vi "Trajectory Builder.vi"() -> ()   [LabVIEW 2023]
uses:
  Types/Limits.ctl
  Types/Overrides.ctl
  Types/Trajectory Data.ctl
  Types/Segment Type.ctl
  Types/Path Type.ctl
  Types/Drive Type.ctl
  Types/Angluar Limits.ctl
  Types/Command Editor Info.ctl
  Types/Single Cmd Info.ctl
  <vilib>/picture/picture.llb/imagedata.ctl
  <vilib>/Utility/miscctls.llb/LVPositionTypeDef.ctl
  <vilib>/Utility/miscctls.llb/LVRowAndColumnTypeDef.ctl
  Types/Internal Path Stuff.ctl
  <vilib>/event_ctls.llb/lveventtype.ctl
  6a65ebb4-e776-4ba2-b94f-6ff829af6114.vi
  6a65ebb4-e776-4ba2-b94f-6ff829af6114.vi/c0db33a9-eb6c-44d9-b982-8563e05d2734.vi
  6a65ebb4-e776-4ba2-b94f-6ff829af6114.vi/ae3535a8-0066-4e8d-a5de-b07ac05a7c65.vi
  6a65ebb4-e776-4ba2-b94f-6ff829af6114.vi/dda8e586-731b-4197-ad83-6a4d05585a0a.vi
  Global Settings.vi
  <vilib>/Utility/cursorutil.llb/Set Cursor (Icon Pict).vi
  <vilib>/Comparison/Less/Less Functor/Less Functor.lvclass
panel:
  in  "Delete":bool
  in  "New Page Selector":T1(radio)
  in  "Push":bool
  out "Picture":picture
  out "RS":bool=TRUE
  in  "Cache":T5
  in  "Zero Velocity":bool
  in  "Reverse Path":bool
  in  "Robot Backwards":bool
  out "Duration (s)":dbl format="%#.4g"
  out "Distance (ft)":dbl format="%#.1g"
  in  "Instructions":string="Directions:\nUse mouse to ...\n    move robot position (rectangle with arrow)\n    rotate robot (red arrow)\n    move waypoints (numbered circles)\nClick in open space to add a waypoint\nShift click to delete a waypoint\nHover over a waypoint and use arrow keys to nudge\n\nTime slider and Play button will run robot along path to test for collisions.\n\nNew creates a new path at default location\n\nAppend creates a path using current path's position and heading.\n\nTo add a command, move robot using Time slider and double click the Command in Palette.\n\nYou can modify command timing in the graph or Command Sequencer tree.\n\nEnable/disable a command by clicking on the enable column item.\n\nDelete a command by shift-clicking in the enable column.\n\nTo configure command parameters, Select the command name in the tree, Open Panel, enter parameters, and Inhale the parameters.\n\nYou may sometimes want to type values into WayPoints directly.\n\nOverrides allow you to set accel and V limits for any turn."
  out "Command Palette":picture
  in  "Directory":bool
  in  "Tab Control":T1(tab)
  in  "Vertical Reflection":bool
  in  "Angular Limits":T6={"Velocity (deg/s)"=6.0, "Accel (deg/s^2)"=360.0, "Jerk (deg/s^3)"=1000.0} {"Jerk (deg/s^3)" min=0.01 step=1.0; "Accel (deg/s^2)" min=0.01; "Velocity (deg/s)" min=0.01}
  in  "Path Type":T7=enum."Bezier"
  in  "Overrides":T8=[{"Count"="1", "Angular Override"=0.0, "Enabled?"=FALSE, "Velocity Override"=6.0, "Angle Override"=nan}] {"Angle Override" step=5.0; "Velocity Override" step=5.0; "Angular Override" step=5.0}
  in  "Horizontal Reflection":bool
  in  "Sample Period (s)":dbl=0.02 min=0.001 max=1.0 format="%#_6p"
  in  "Limits":T9={"Velocity (fps)"=6.0, "Accel (fps^2)"=15.0, "Jerk (fps^3)"=150.0, "StoopidFast (fps)"=6.0} {"StoopidFast (fps)" min=0.01; "Jerk (fps^3)" min=0.01 step=1.0; "Accel (fps^2)" min=0.01; "Velocity (fps)" min=0.01}
  in  "Conditions":T10 {"vFinal (fps)" min=0.0; "vInitial (fps)" min=0.0}
  in  "Drive Type":T11
  in  "Turn Rate":dbl=5.0 format="%#_13g"
  in  "WayPoints":cluster{"x":dbl, "y":dbl, "th":dbl}[](array[cluster])
  in  "Turn Angle Limit (deg)":dbl=90.0
  in  "Allow Angles > 90":bool=TRUE
  in  "Stoopid Overlap %":dbl min=0.0
  in  "Unjank":bool
  in  "Turn Deceleration":bool=TRUE
  in  "Turn Acceleration":bool=TRUE
  out "Trajectory Data":T12
  in  "Open Command":bool
  in  "Inhale":bool
  in  "Command Sequence":string(tree)
  in  "Projects":u16(ring) items=["Reefscape.lvproj"]
  in  "Refresh":bool
  in  "Snap to foot":bool
  in  "Angle Limiter":enum16{"90", "45", "15", "1"}(ring)=enum."15"
  in  "Snap robot to baseline":bool
  in  "Background":u16(ring) items=["RS Field"]
  in  "Robot Color":u32(colorbox)=14421504
  out "Field Size (ft)":cluster{"width":dbl, "height":dbl}={"width"=26.4166, "height"=57.5729} {"width" format="%#.1g"; "height" format="%#.1g"}
  in  "Robot Size (in)":cluster{"width":dbl, "height":dbl}={"width"=37.0, "height"=32.0}
  in  "Hide Path":bool
  in  "Time (s)":dbl(slide) scale=0.0..3.9399999119341373 scale format="%#.1g"
  in  "Play":bool
  out "fps":dbl[](graph)
  in  "Append":bool
  in  "Open":i32[](listbox)
  in  "Filename":string
  in  "Save":bool
  in  "New":bool
  # "Command Palette"
  # "StupidFast makes each linear segment into a\nvelocity ramp to max speed (for clothoid paths only)"
  # "Nicotine"
  # "A"
  # "V"
  # "O"
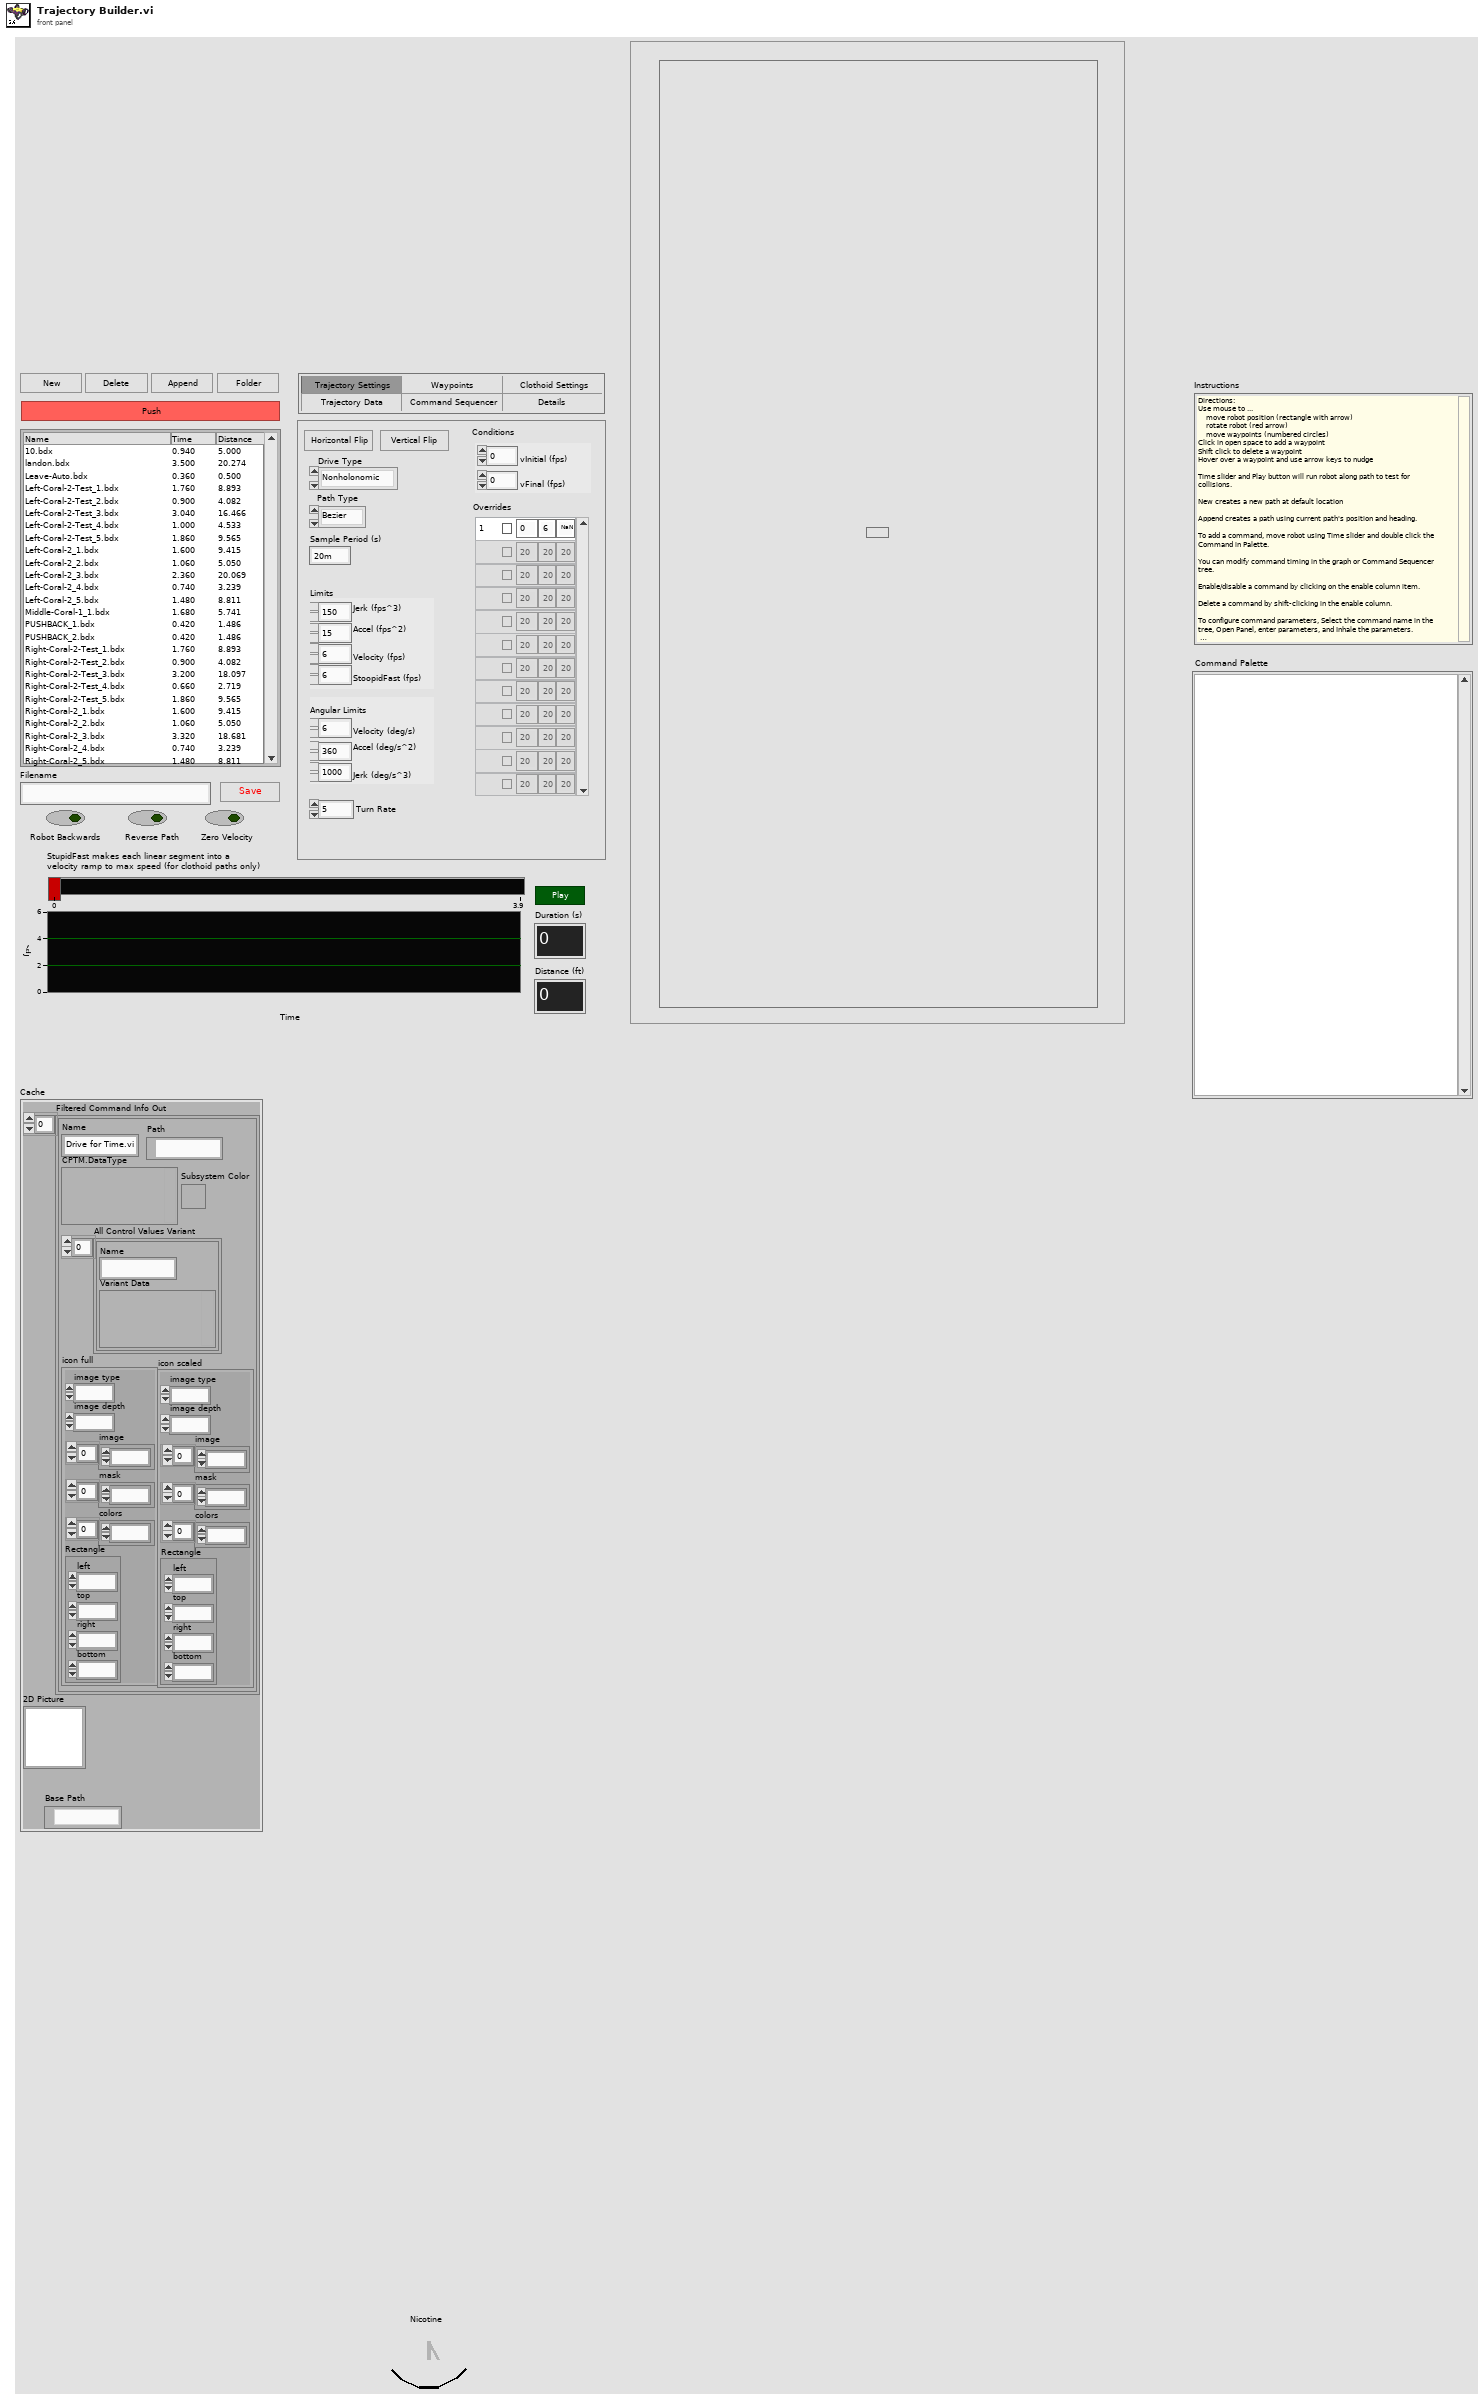
[diagram p1: front panel]
types:
  T1 = enum32{"Trajectory Settings", "Waypoints", "Clothoid Settings", "Trajectory Data", "Command Sequencer", "Details"}
  T2 = typedef "Command Editor Info.ctl" = T3[]
  T3 = typedef "Single Cmd Info.ctl" = cluster{"Name":string, "CPTM.DataType":variant, "All Control Values Variant":cluster{"Name":string, "Variant Data":variant}[], "icon full":T4, "icon scaled":T4, "Path":path, "Subsystem Color":u32}
  T4 = typedef "imagedata.ctl" = cluster{"image type":i32, "image depth":i32, "image":u8[], "mask":u8[], "colors":u32[], "Rectangle":cluster{"left":i16, "top":i16, "right":i16, "bottom":i16}}
  T5 = cluster{"Filtered Command Info Out":T2, "2D Picture":picture, "Base Path":path}
  T6 = typedef "Angluar Limits.ctl" = cluster{"Velocity (deg/s)":dbl, "Accel (deg/s^2)":dbl, "Jerk (deg/s^3)":dbl}
  T7 = typedef "Path Type.ctl" = enum16{"Clothoid", "Bezier"}
  T8 = typedef "Overrides.ctl" = cluster{"Count":string, "Angular Override":dbl, "Enabled?":bool, "Velocity Override":dbl, "Angle Override":dbl}[]
  T9 = typedef "Limits.ctl" = cluster{"Velocity (fps)":dbl, "Accel (fps^2)":dbl, "Jerk (fps^3)":dbl, "StoopidFast (fps)":dbl}
  T10 = cluster{"vInitial (fps)":dbl, "vFinal (fps)":dbl}
  T11 = typedef "Drive Type.ctl" = enum16{"Nonholonomic", "Holonomic"}
  T12 = typedef "Trajectory Data.ctl" = cluster{"Segment Name":string, "Type":T13, "Traj Pos Points":cluster{"x":dbl, "y":dbl, "th":dbl}[], "Traj Vel Points":cluster{"V":dbl, "Omega":dbl, "V vector":cluster{"y":dbl, "x":dbl}}[], "Accel Index":i32, "Decel Index":i32}[]
  T13 = typedef "Segment Type.ctl" = enum16{"Accel Straight", "Const Straight", "Blend", "Circle", "Bezier"}
  T14 = cluster{"Sample Period (s)":dbl, "Limits":T9, "Conditions":cluster{"vInitial (fps)":dbl, "vFinal (fps)":dbl}, "Overrides":T8, "Angular Limits":T6}
  T15 = typedef "LVRowAndColumnTypeDef.ctl" = cluster{"Row":i32, "Column":i32}
  T16 = typedef "LVPositionTypeDef.ctl" = cluster{"Left":i32, "Top":i32}
  T17 = cluster{"Index":i32, "Pt Test Results":enum16{"Miss", "Rect Hit", "Arrow Hit"}}
  T18 = cluster{"Drag Object":cluster{"Index":i32, "x":dbl, "y":dbl}, "Hover Object":cluster{"Index":i32, "Pt Test Results":enum16{"Miss", "Rect Hit", "Arrow Hit"}}, "Filename":string}
  T19 = cluster{"Trajectory Data":T12, "Points":cluster{"x":dbl, "y":dbl, "th":dbl}[], "output cluster":cluster{"Sample Period (s)":dbl, "Limits":T9, "Conditions":cluster{"vInitial (fps)":dbl, "vFinal (fps)":dbl}, "Overrides":T8, "Angular Limits":T6}, cluster{"Time (s)":dbl, T3, bool}[]}
  T20 = typedef "Internal Path Stuff.ctl" = cluster{"Trajectory Data":T12, "Updated Waypoints":cluster{"x":dbl, "y":dbl, "th":dbl}[], cluster{"Sample Period (s)":dbl, "Limits":T9, "Conditions":cluster{"vInitial (fps)":dbl, "vFinal (fps)":dbl}, "Overrides":T8, "Angular Limits":T6}, "Commands out":cluster{"Time (s)":dbl, T3, bool}[]}
  T21 = typedef "lveventtype.ctl" = enum32{"Null", "Timeout", "Annotation Menu Selection", "Annotation Menu Selection?", "App Instance Close", "App Instance Close?", "Autoscale Range Change", "Bookmark Info Change", "Cell Edit", "Cell Edit?", "Cursor Grab", "Cursor Grab?", "Cursor Menu Selection", "Cursor Menu Selection?", "Cursor Move", "Cursor Release", "Data Change", "Direction Change", "Display State Change", "Drag Ended", "Drag Enter", "Drag Leave", "Drag Over", "Drag Source Update", "Drag Starting", "Drag Starting?", "Drop", "Exec State Change", "Key Down", "Key Down?", "Key Repeat", "Key Repeat?", "Key Up", "Listbox Double Click", "Menu Activation?", "Menu Selection (App)", "Menu Selection? (App)", "Menu Selection (User)", "Mouse Down", "Mouse Down?", "Mouse Enter", "Mouse Leave", "Mouse Move", "Mouse Up", "Mouse Wheel", "NI Security User Change (App)", "Pane Size", "Panel Close", "Panel Close?", "Panel Resize", "Plot Attribute Change", "Scale Range Change", "Shortcut Menu Activation?", "Shortcut Menu Selection (App)", "Shortcut Menu Selection? (App)", "Shortcut Menu Selection (User)", "Tree Double Click", "Tree Drag", "Tree Drag?", "Tree Drop", "Tree Drop?", "Tree Item Close", "Tree Item Close?", "Tree Item Open", "Tree Item Open?", "User Event", "Value Change"}
  T22 = enum32{"Invalid", "Standard", "Closed", "Hidden", "Minimized", "Maximized"}
  T23 = cluster{"width":dbl, "height":dbl, "width":dbl, "height":dbl}
  T24 = cluster{"status":bool, "code":bool, "source":bool}
  T25 = cluster{"Robot Backwards":bool, "Reverse Path":bool}
  T26 = cluster{cluster{"Robot Backwards":bool, "Reverse Path":bool}, "Trajectory Data":T12, "sorted array out":cluster{"Time (s)":dbl, T3, bool}[], cluster{"Sample Period (s)":dbl, "Limits":T9, "Conditions":cluster{"vInitial (fps)":dbl, "vFinal (fps)":dbl}, "Overrides":T8, "Angular Limits":T6}, "Updated Waypoints":cluster{"x":dbl, "y":dbl, "th":dbl}[], cluster{"Time (s)":dbl, "Distance (ft)":dbl}, "Zero Velocity":bool, cluster{"Drive Type":T11, "Path Type":T7}}
  T27 = cluster{"Trajectory Data":T12, "Updated Waypoints":cluster{"x":dbl, "y":dbl, "th":dbl}[], cluster{"Sample Period (s)":dbl, "Limits":T9, "Conditions":cluster{"vInitial (fps)":dbl, "vFinal (fps)":dbl}, "Overrides":T8, "Angular Limits":T6}, "sorted array out":cluster{"Time (s)":dbl, T3, bool}[]}
  T28 = cluster{"Sample Period (s)":dbl, cluster{"Velocity (fps)":dbl, "Accel (fps^2)":dbl, "Jerk (fps^3)":dbl, "StoopidFast (fps)":dbl}, "Conditions":cluster{"vInitial (fps)":dbl, "vFinal (fps)":dbl}, "Overrides":T8, "Angular Limits":T6}
  T29 = cluster{"Velocity (fps)":dbl, "Accel (fps^2)":dbl, "Jerk (fps^3)":dbl, "StoopidFast (fps)":dbl}
  T30 = cluster{"Trajectory Data":T12, "Points out":cluster{"x":dbl, "y":dbl, "th":dbl}[], "Fields":cluster{"Sample Period (s)":dbl, cluster{"Velocity (fps)":dbl, "Accel (fps^2)":dbl, "Jerk (fps^3)":dbl, "StoopidFast (fps)":dbl}, "Conditions":cluster{"vInitial (fps)":dbl, "vFinal (fps)":dbl}, "Overrides":T8, "Angular Limits":T6}, "Commands out":cluster{"Time (s)":dbl, T3, bool}[]}
  T31 = typedef "LVPoint32TypeDef.ctl" = cluster{"Horizontal":i32, "Vertical":i32}
  T32 = cluster{"Shift":bool, "Ctrl":bool, "Alt":bool, "Cmd":bool, "Opt":bool}
  T33 = typedef "LVBoundsTypeDef.ctl" = cluster{"Width":u32, "Height":u32}
  T34 = cluster{"Snap robot to baseline":bool, "Snap to foot":bool, "Angle Limiter":enum16{"90", "45", "15", "1"}}
  T35 = cluster{i32, "Pt Test Results":enum16{"Miss", "Rect Hit", "Arrow Hit"}}
  T36 = typedef "eventvkey.ctl" = enum16{"ASCII", "Enter", "Return", "Shift", "Ctrl", "Alt", "Cmd", "Opt", "Caps", "NumLock", "Clear", "Break", "Up", "Down", "Left", "Right", "Insert", "Delete", "Home", "End", "PageUp", "PageDown", "Escape", "Help", "Pause", "ScrollLock", "F1", "F2", "F3", "F4", "F5", "F6", "F7", "F8", "F9", "F10", "F11", "F12", "F13", "F14", "F15", "F16", "F17", "F18", "F19", "F20", "F21", "F22", "F23", "F24", "Play", "VolumeUp", "VolumeDown", "Mute", "Two Byte Char"}
  T37 = cluster{"Name":string, "CPTM.DataType":variant, "Get All Control Values Variant":cluster{"Name":string, "Variant Data":variant}[], "Color 256":T4, "Subsystem Color":u32}[]
  T38 = cluster{"Filtered Command Info Out":T2, "2D Picture":picture, "stripped path":path}
  T39 = cluster{"Horizontal":dbl, "Vertical":dbl, "th":dbl}
  T40 = cluster{"Name":string, "Color":u32, "Style":i32, "Point Style":i32, "Name Visible":bool, "Allow Drag":bool, "Annotation Mode":i32, "Plot":i32, "Index":i32, "Position":cluster{"X":dbl, "Y":dbl}, "X Scale":i32, "Y Scale":u32, "Show Arrow":bool, "Lock Name":bool, "Plot Area":i32, "Label Offset":cluster{"X":dbl, "Y":dbl}}[]
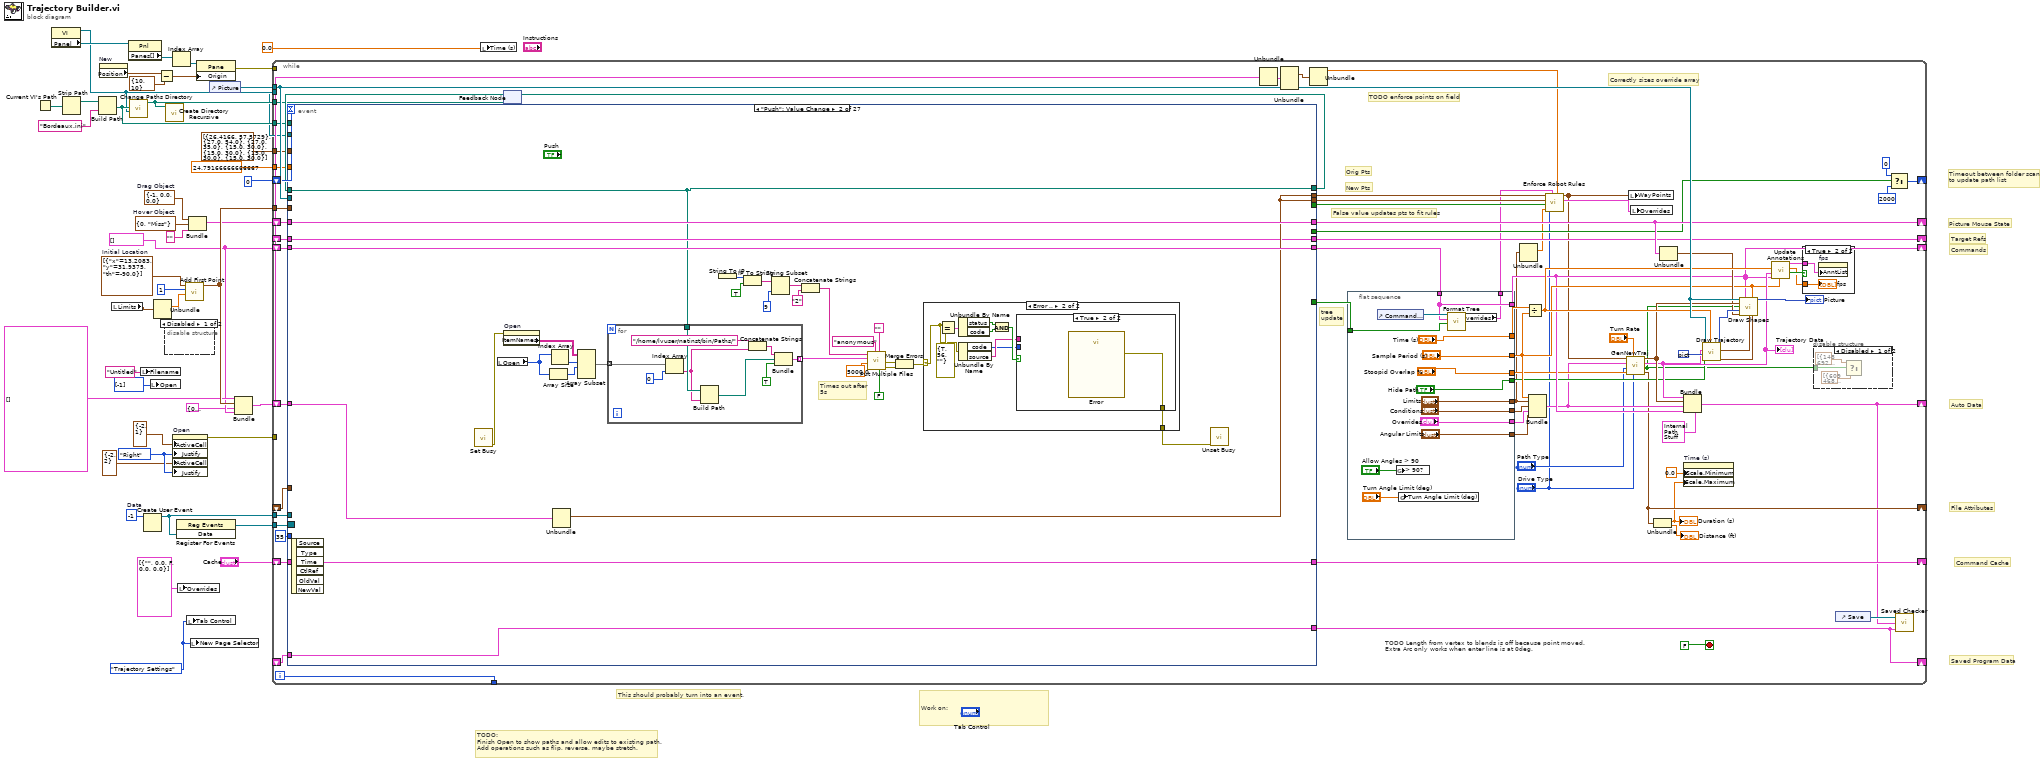
[diagram p0: block diagram]
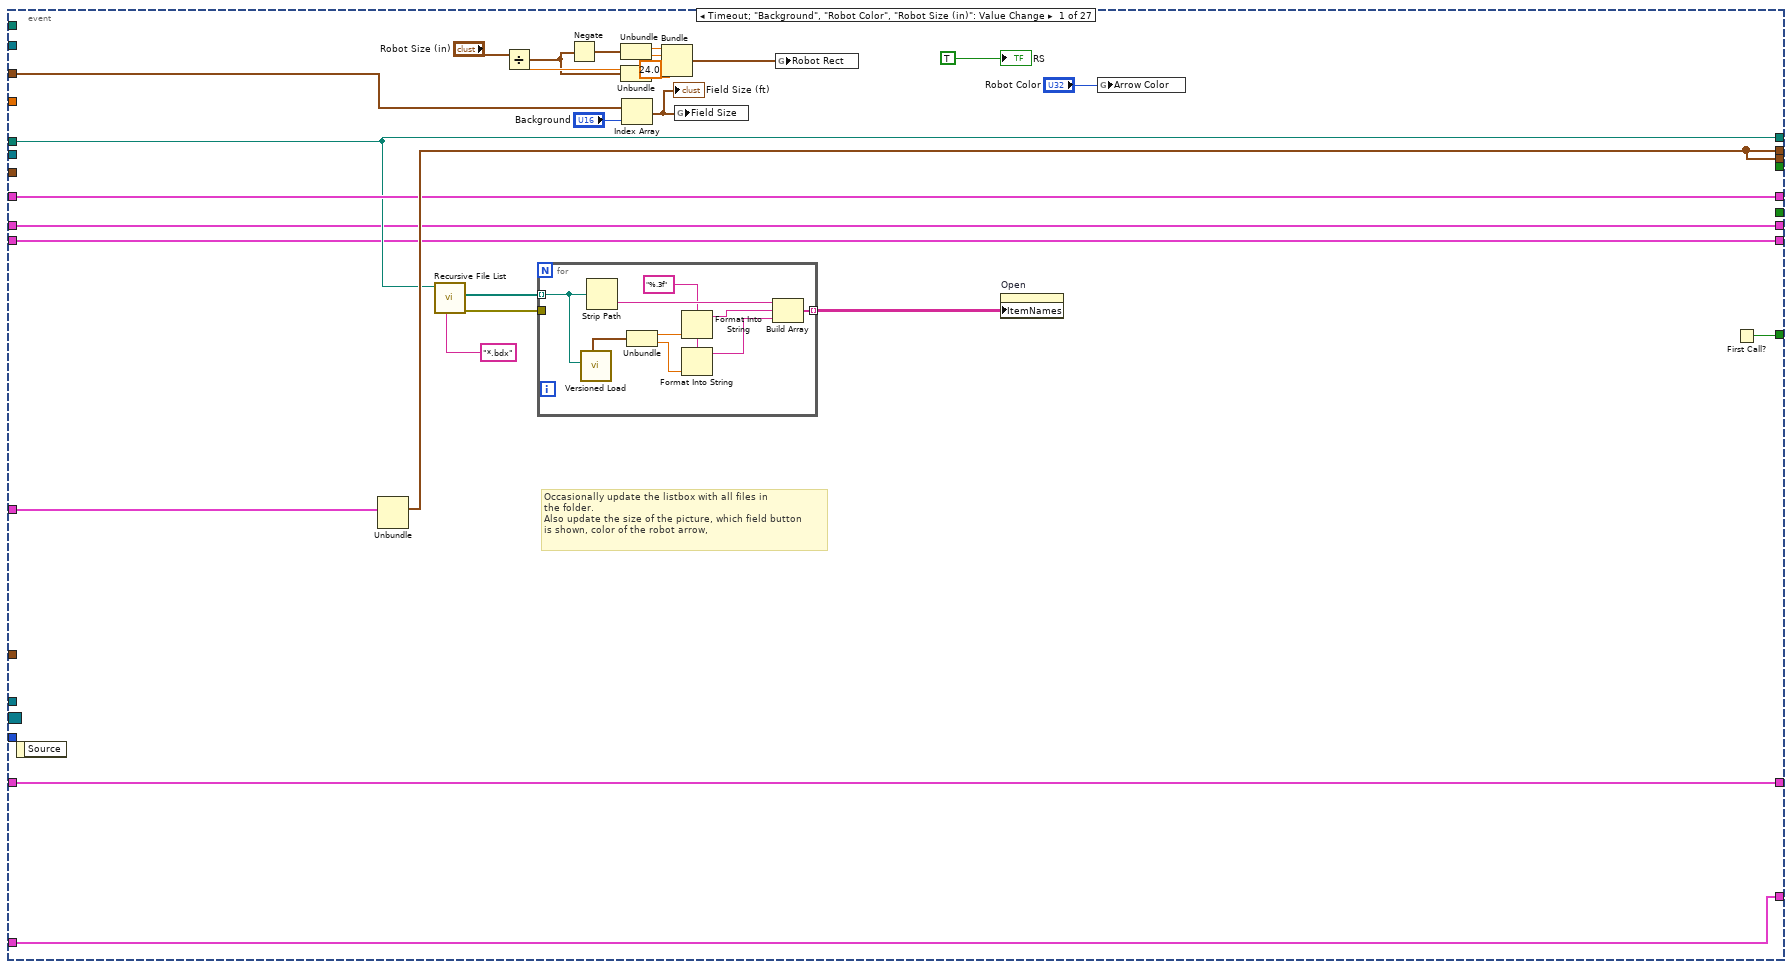
[diagram p4: hidden frame]
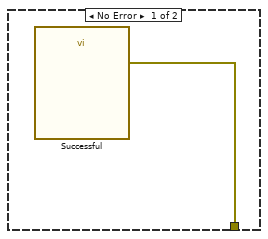
[diagram p5: hidden frame]
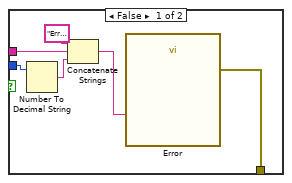
[diagram p6: hidden frame]
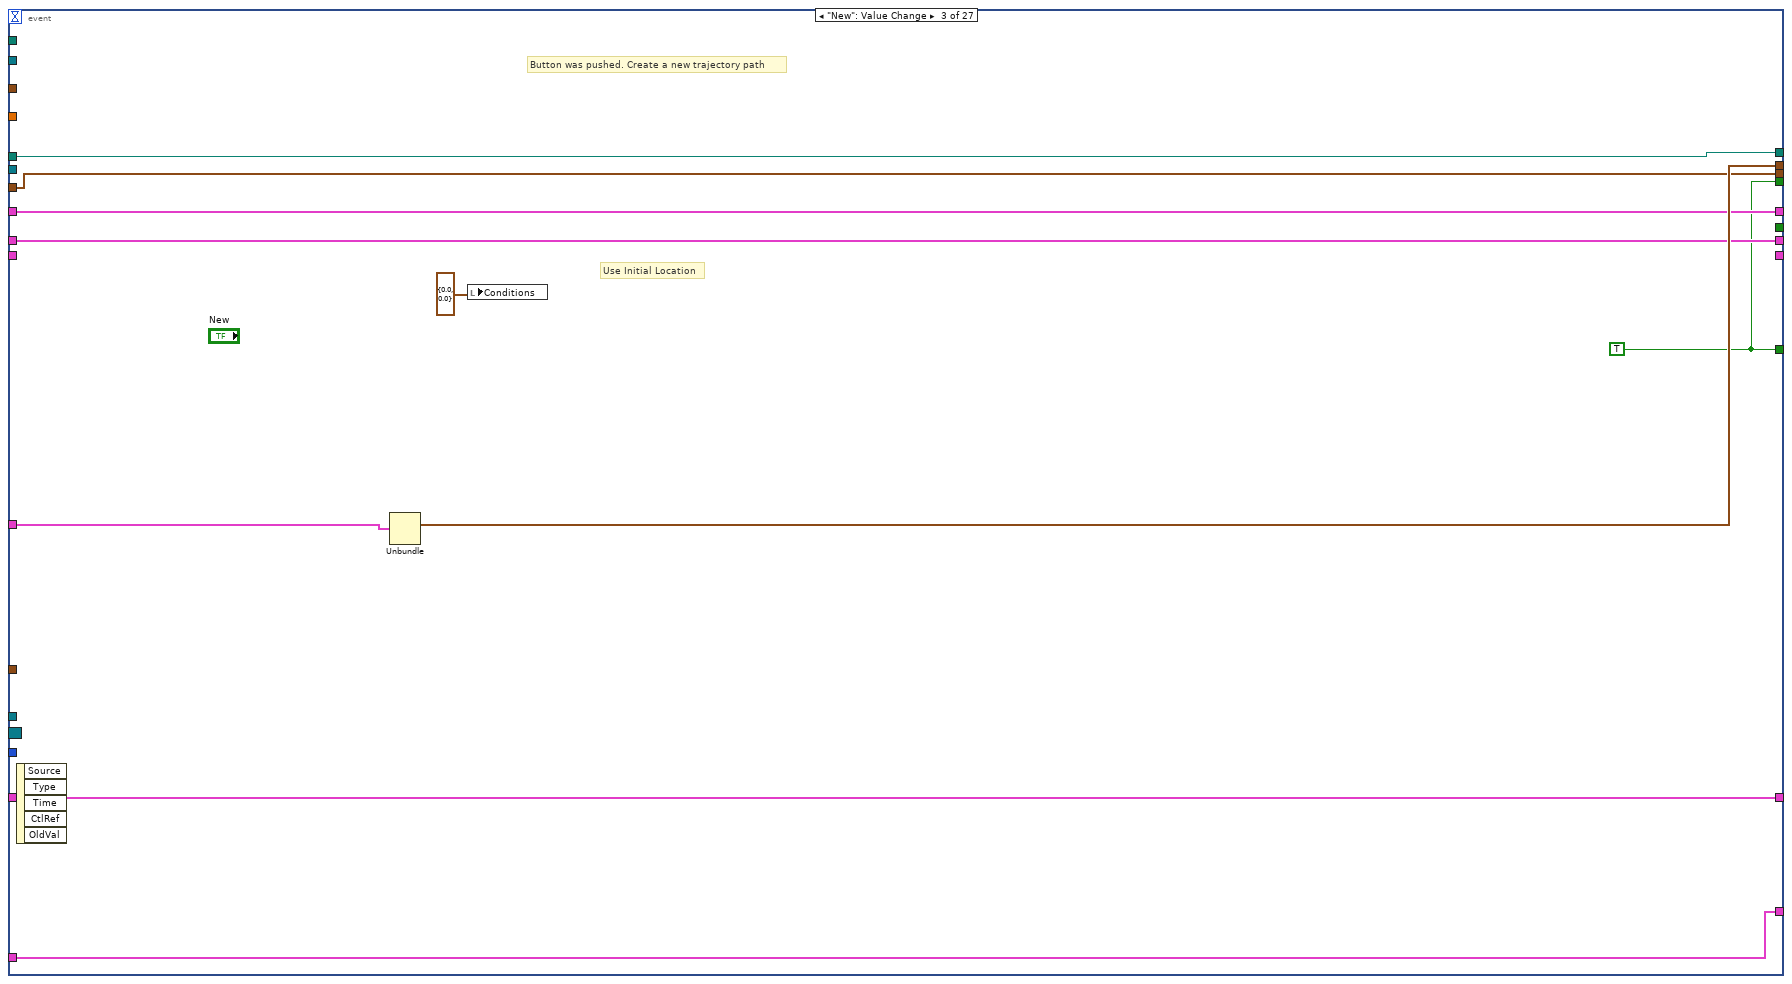
[diagram p7: hidden frame]
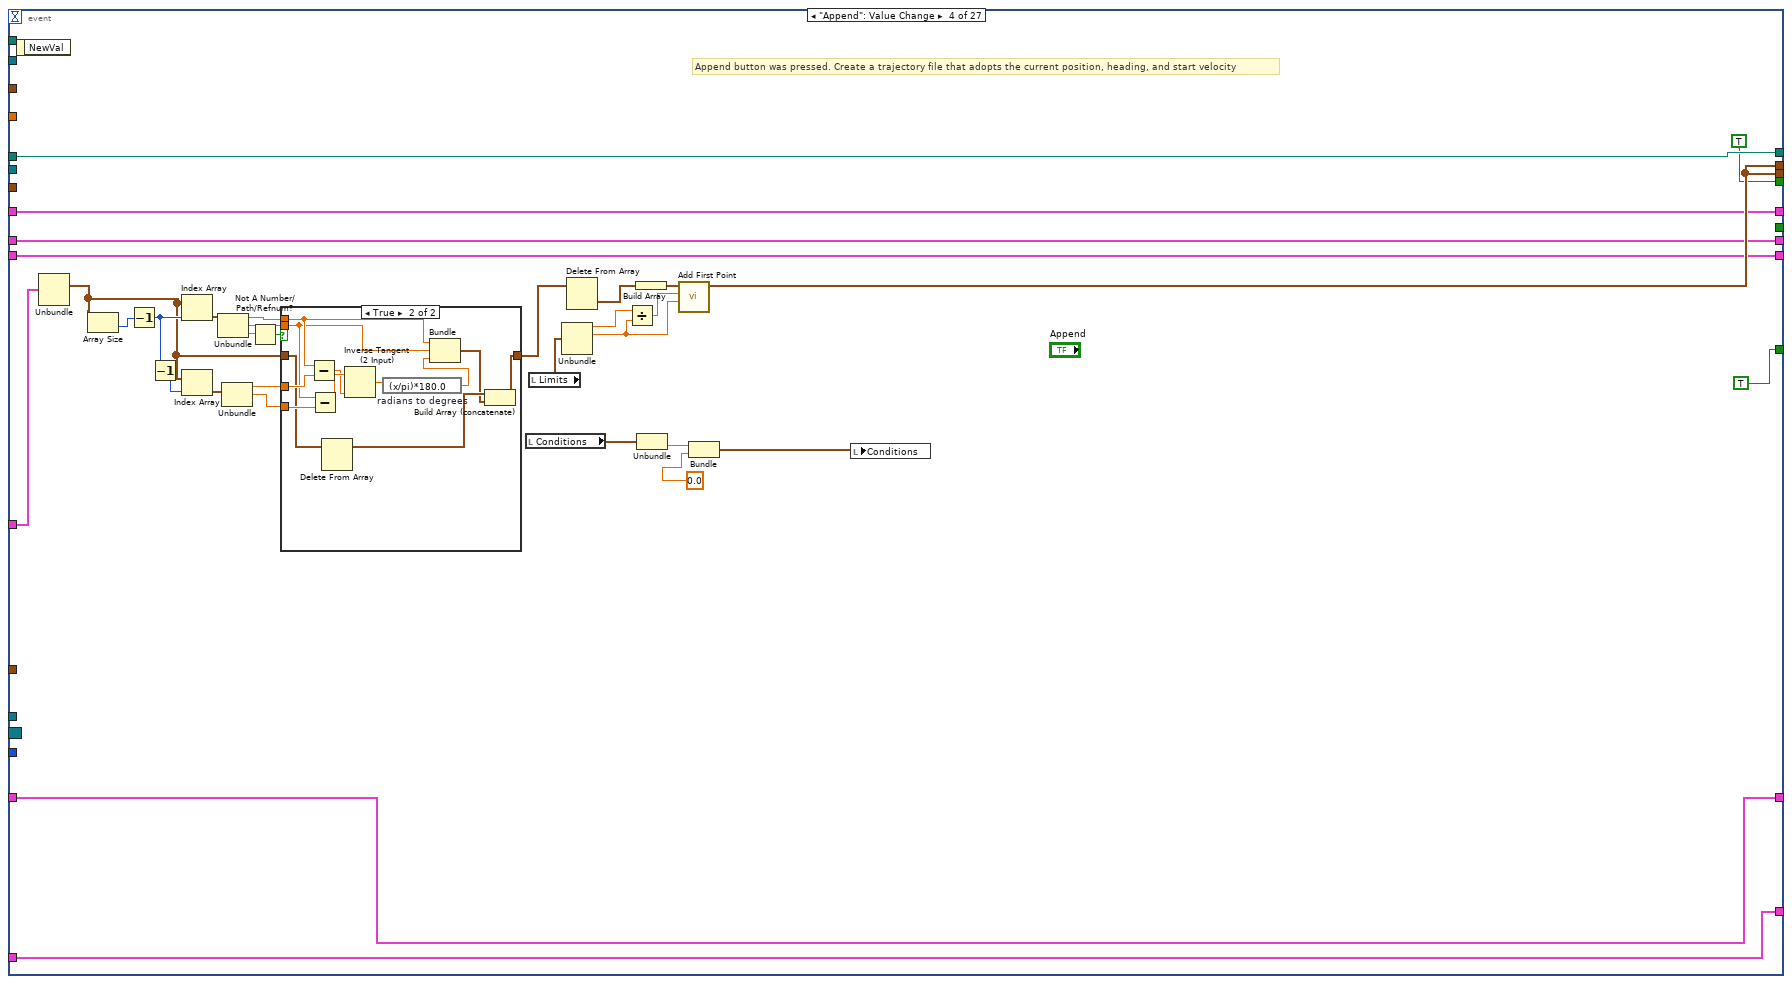
[diagram p8: hidden frame]
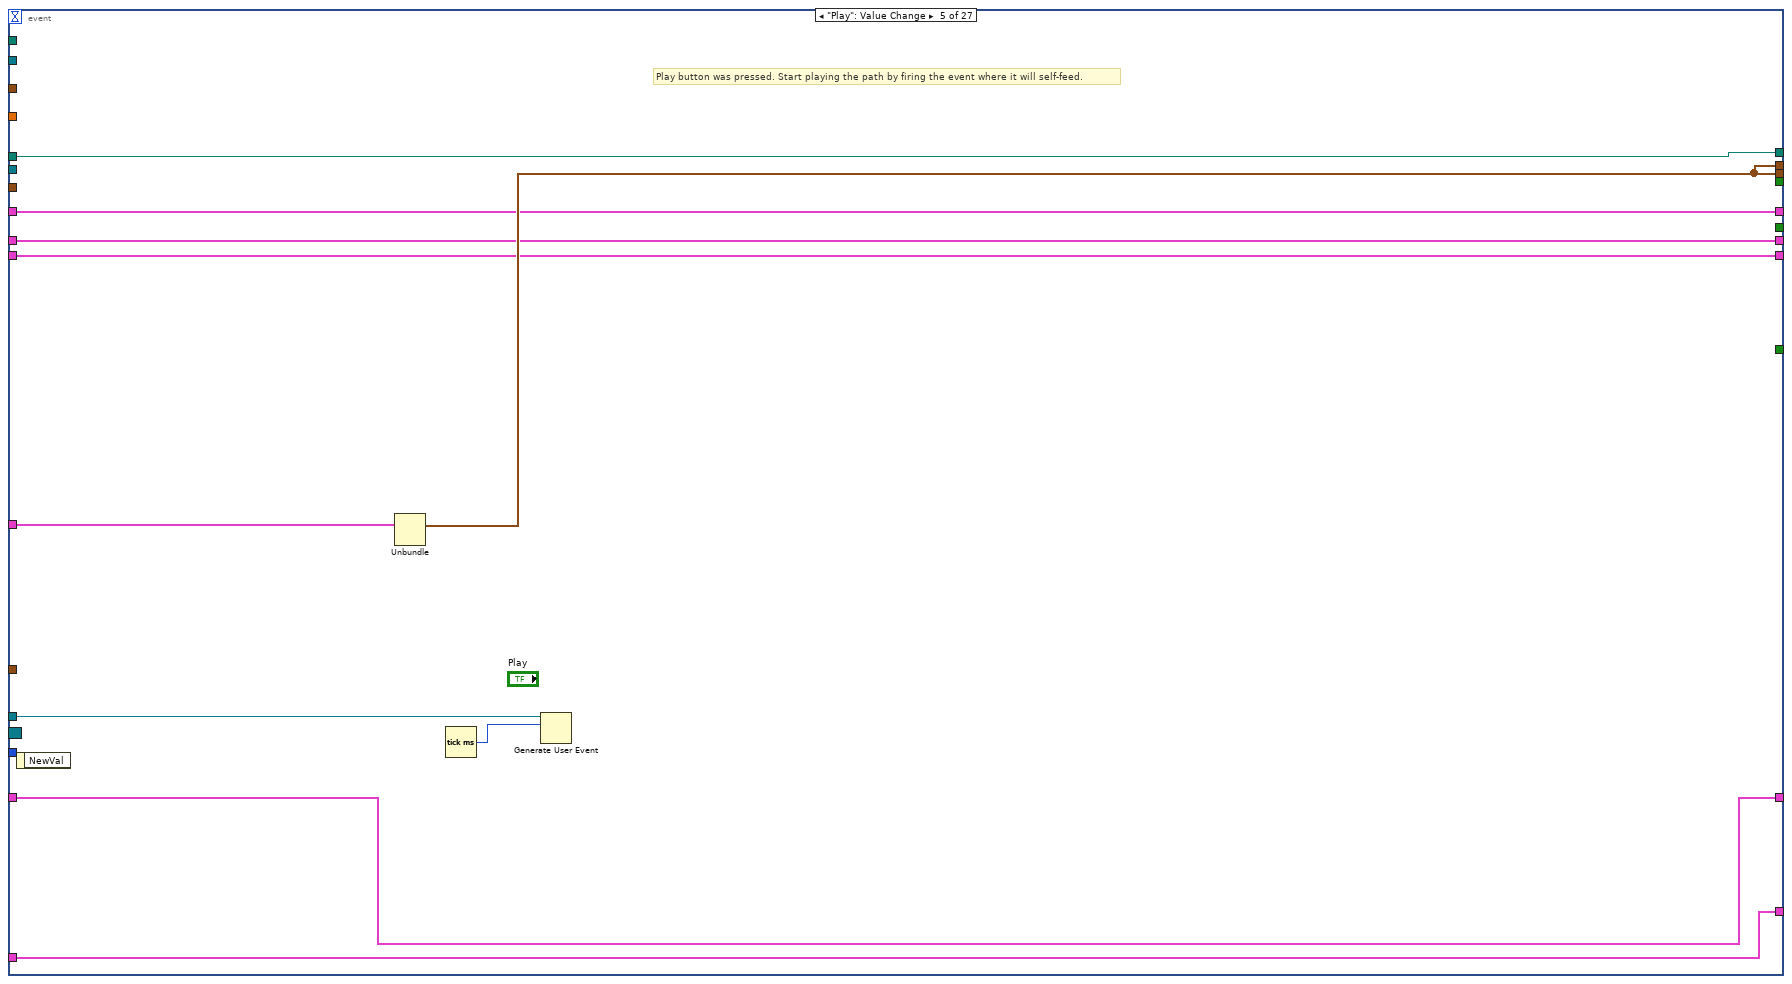
[diagram p10: hidden frame]
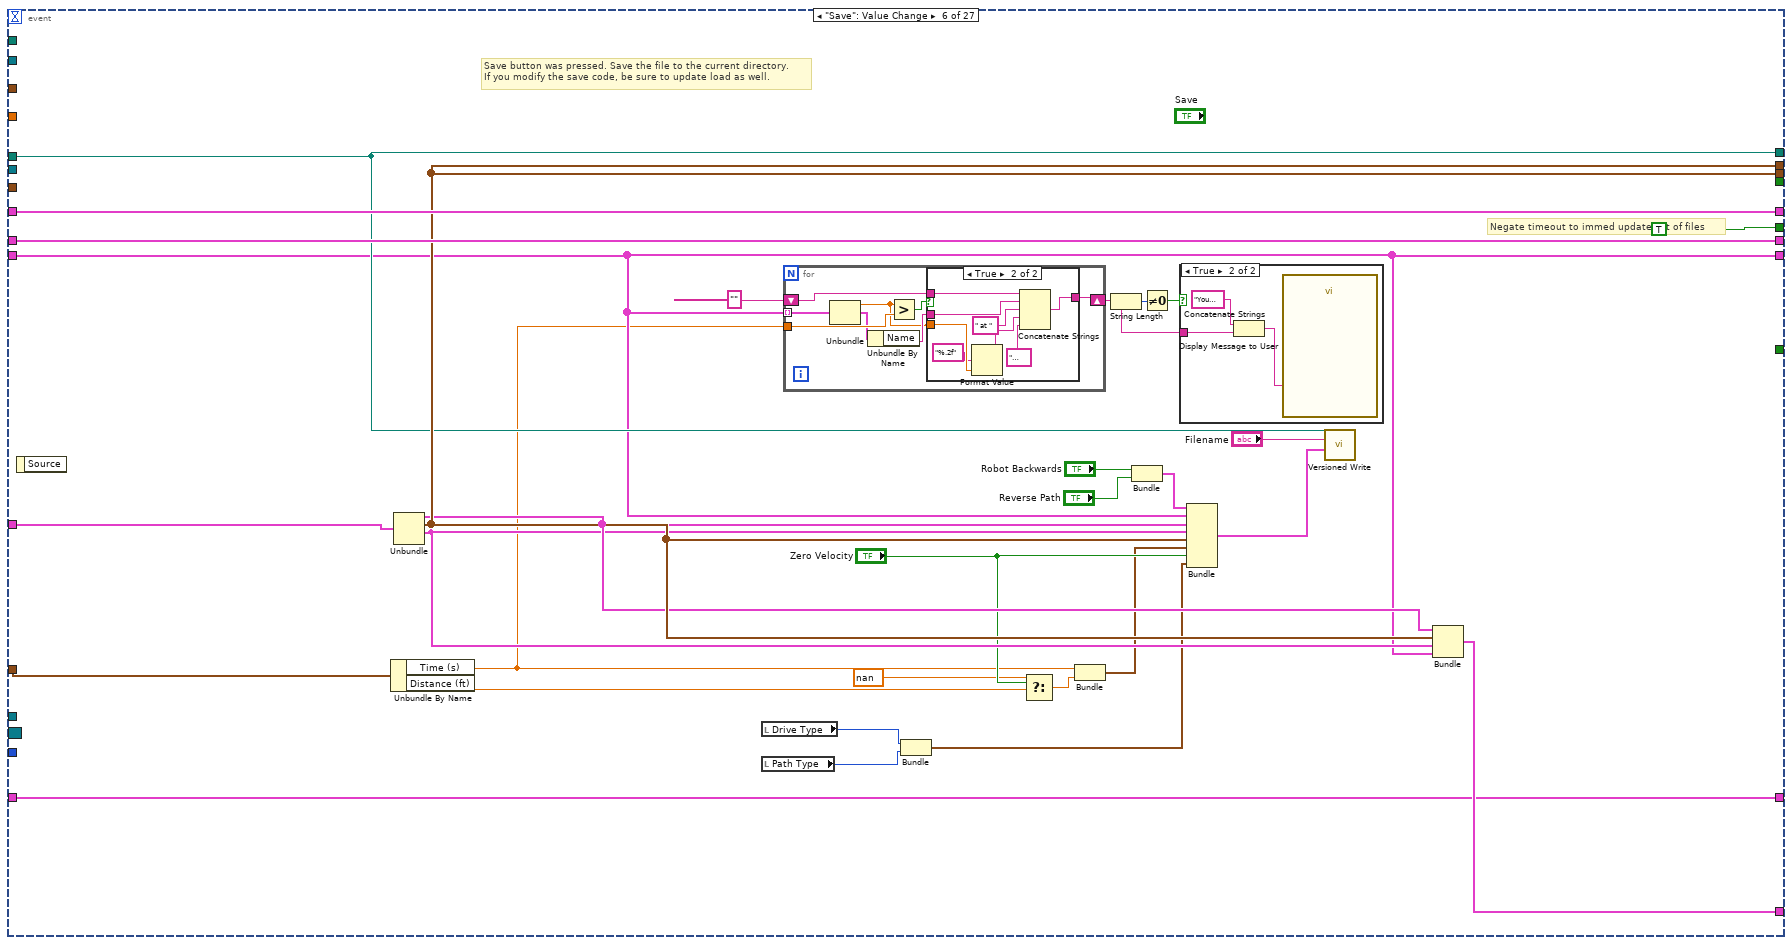
[diagram p11: hidden frame]
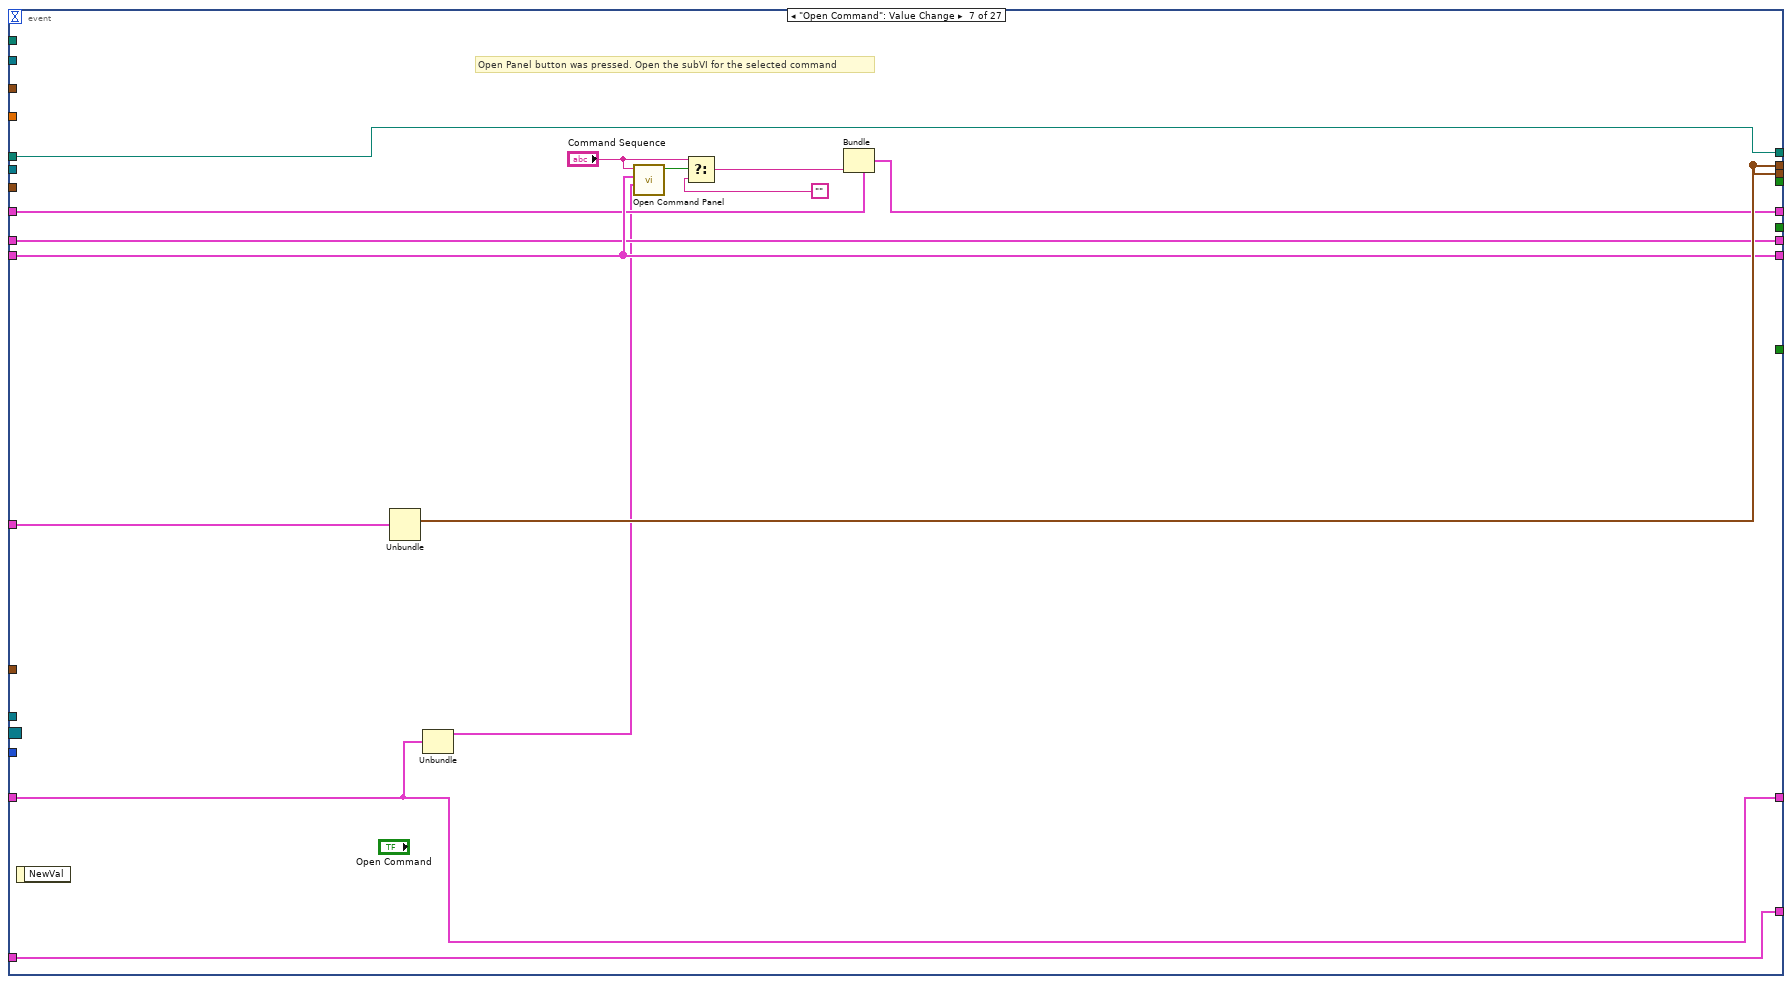
[diagram p14: hidden frame]
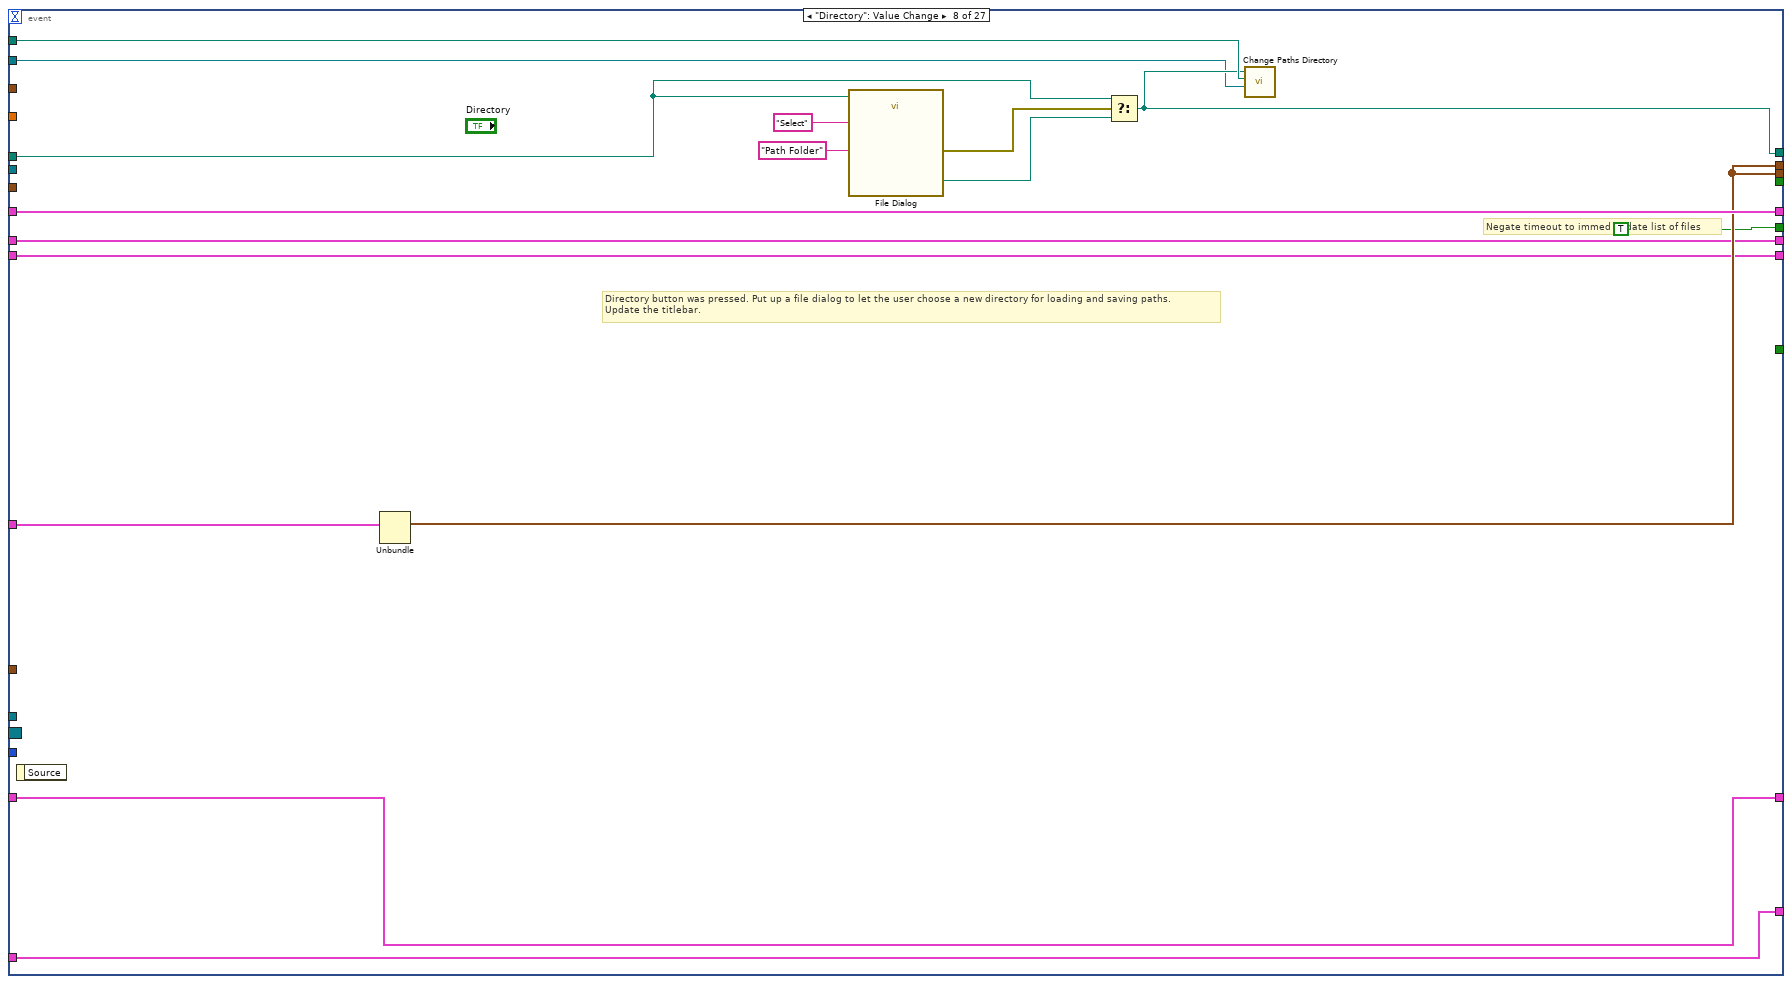
[diagram p15: hidden frame]
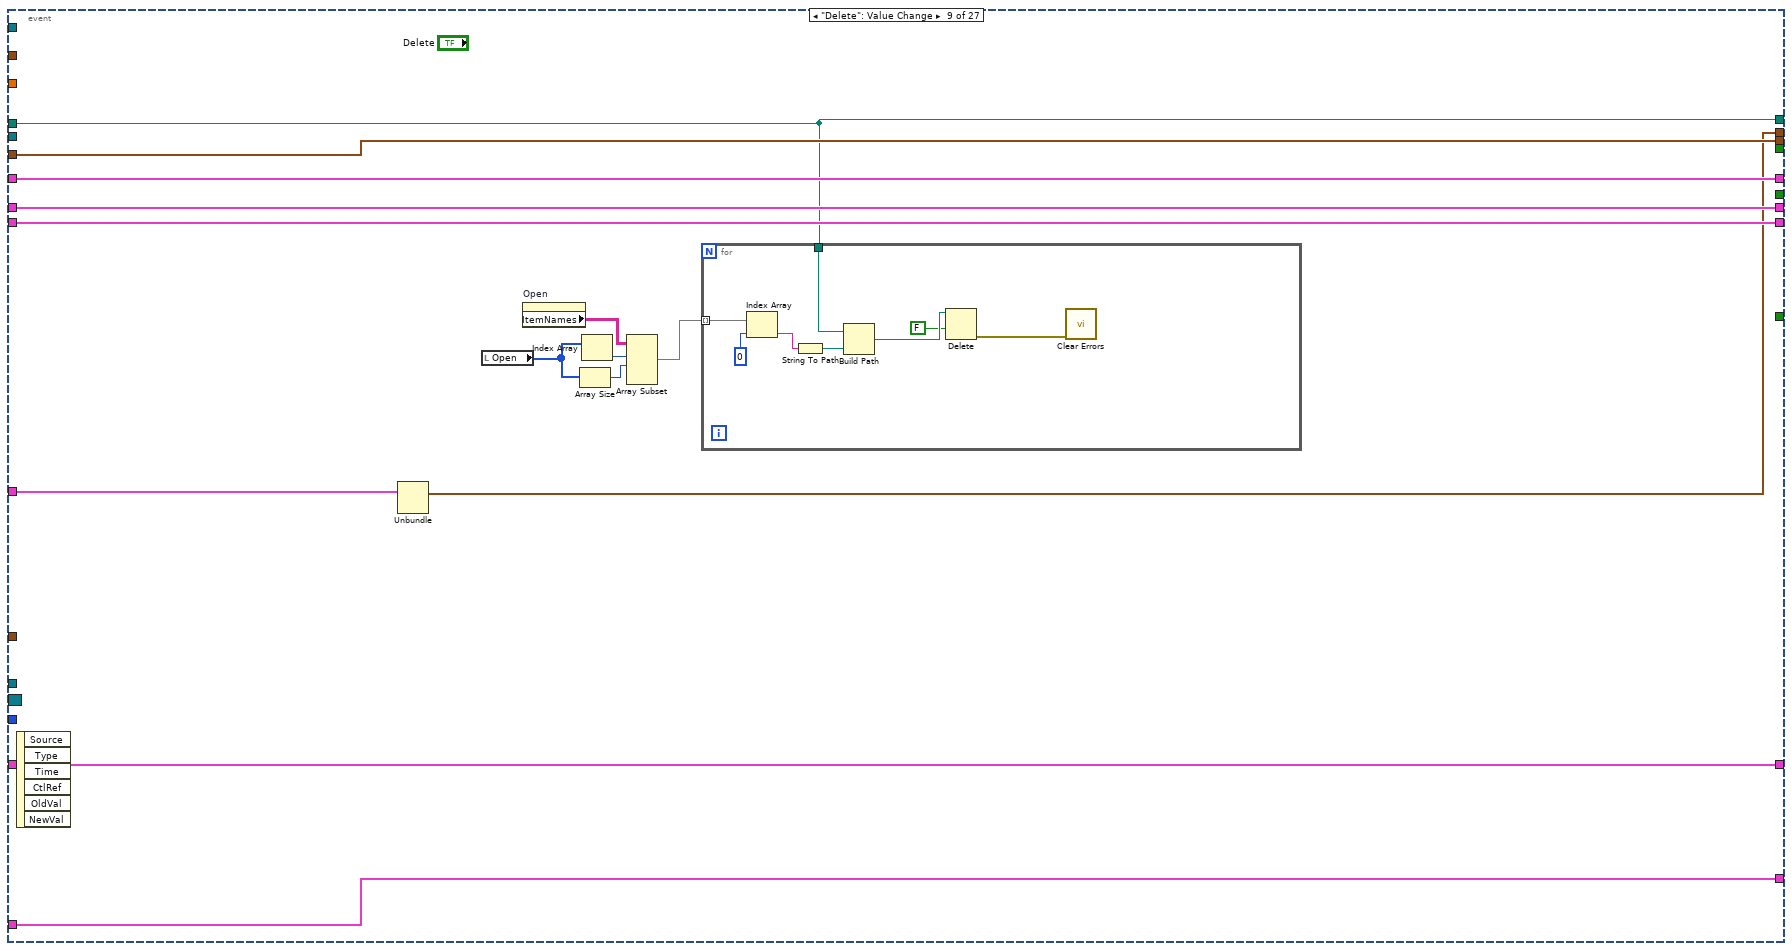
[diagram p16: hidden frame]
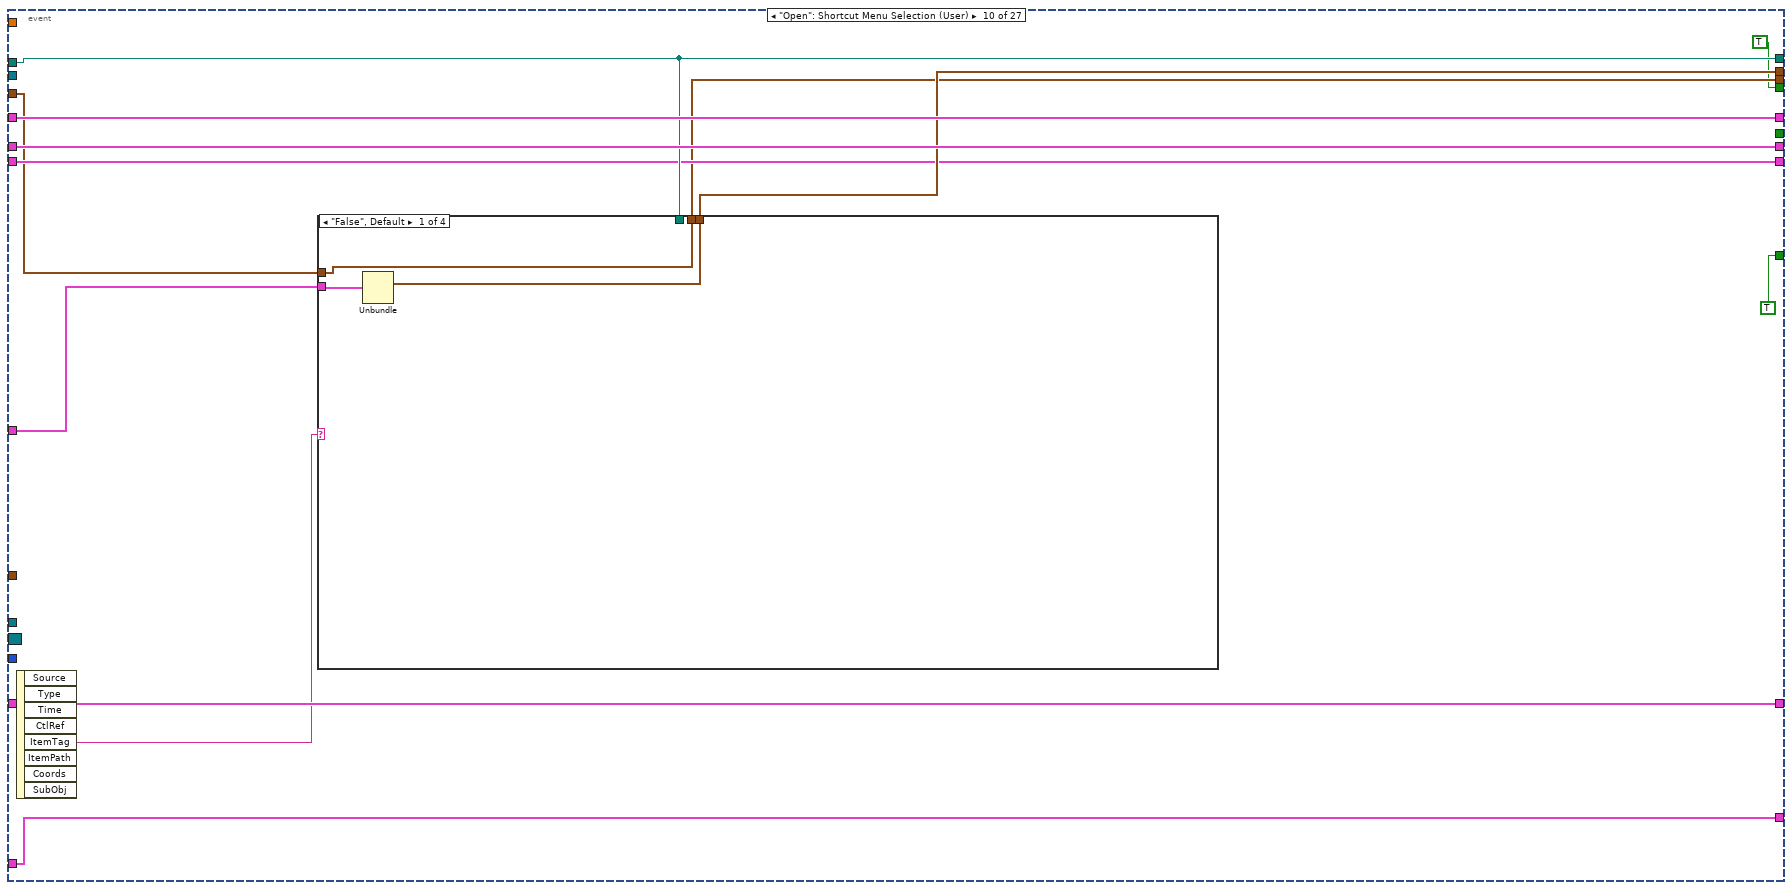
[diagram p17: hidden frame]
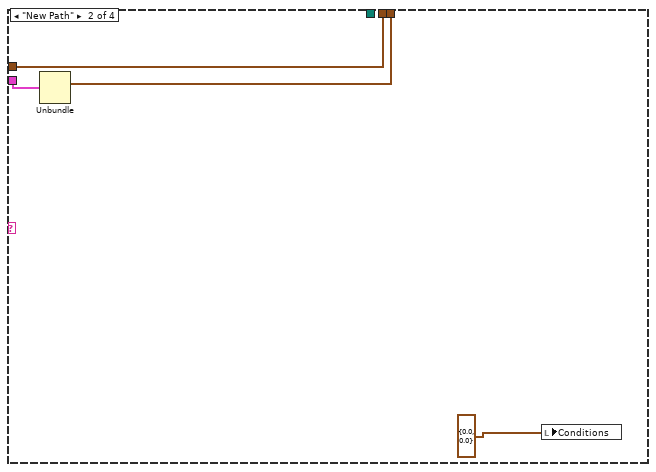
[diagram p18: hidden frame]
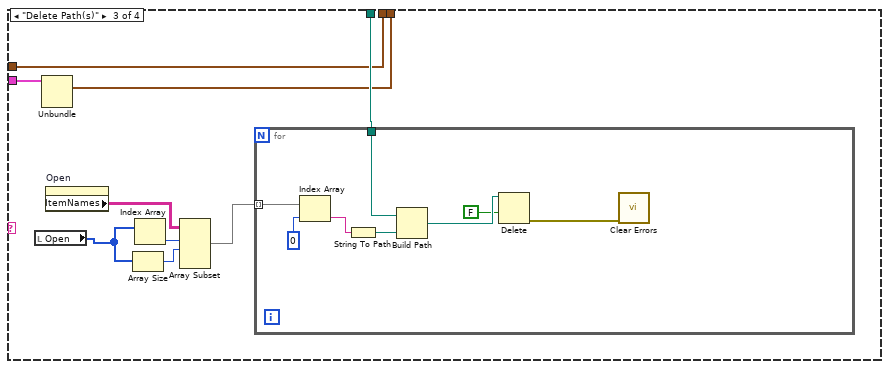
[diagram p19: hidden frame]
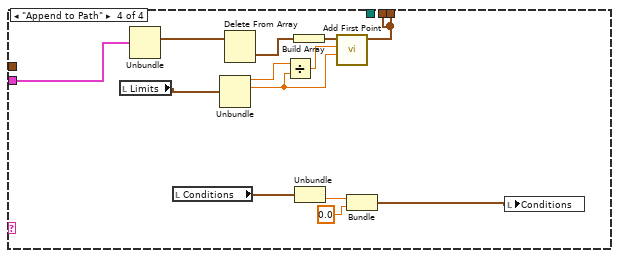
[diagram p20: hidden frame]
diagram:
  w3 = T1."Trajectory Settings" ("Tab Control")
  w12 = enum16{"Left", "Center", "Right"}."Right" ("Active Cell:Cell Justification")
  w19 = cluster{"Time (s)":dbl, T3, bool}[] []
  w33 = -1  # Data
  w30 = T17 {"Index"=0, "Pt Test Results"=enum."Miss"}  # Hover Object
  w29 = cluster{"Index":i32, "x":dbl, "y":dbl} {"Index"=-1, "x"=0.0, "y"=0.0}  # Drag Object
  w41 = cluster{"x":dbl, "y":dbl, "th":dbl}[] [{"x"=13.2083, "y"=31.9375, "th"=-90.0}]  # Initial Location
  # "Saved Program Data"
  # "Command Cache"
  # "File Attributes"
  # "Commands"
  # "Target Refs"
  # "Picture Mouse State"
  # "Auto Data"
  # "Timeout between folder scan\nto update path list"
  # "This should probably turn into an event."
  # "Work on:"
  # "TODO: \nFinish Open to show paths and allow edits to existing path.\nAdd operations such as flip, reverse, maybe stretch."
  n1 = Current VI's Path() -> (path=w17:path)
  n2 = property class="VI"() -> (reference out=w8:refnum<vi>, "Panel"=w27:refnum<vi>)  [unwired: 2 in, 1 out]
  n3 = Strip Path(path=w17) -> (stripped path=w16:path)  [unwired: 1 out]
  n4 = Build Path(base path=w16, name or relative path="Bordeaux.ini" ("format string")) -> (appended path=w10:path)
  n5 = property on="New" class="Bool"() -> ("Position"=w23:T16)  [unwired: 2 in, 2 out]
  n6 = local read "Limits"() -> (w38:T9)
  n7 = property class="Pnl"(reference=w27) -> ("Panes[]"=w26:refnum<vi>[])  [unwired: 1 in, 2 out]
  n8 = call "Change Paths Directory.vi"("VI Refnum"=w8, "config path"=w10) -> ("Bordeaux paths out"=w9:path)  [unwired: 9 in]
  n9 = local write "Filename"("Untitled" ("Filename")) -> ()
  n10 = Create User Event(user event datatype=w33) -> (user event=w34:refnum<user-event>)  [unwired: 1 in, 1 out]
  n11 = local write "Open"(i32[] [-1] ("Open")) -> ()
  n12 = Unbundle(w38) -> ("Accel (fps^2)"=w37:dbl)  [unwired: 3 out]
  n13 = Subtract(x=w23, y=T16 {"Left"=10, "Top"=10}) -> (x-y=w22:T16)
  n14 = disable-structure shown="Disabled" {
    frame Disabled {
    }
    frame Enabled {
    }
  }
  n15 = call <vilib>:"Create Directory Recursive.vi"("directory"=w9) -> ()  [unwired: 4 in, 3 out]
  n16 = Index Array(array=w26) -> (element=w25:refnum<vi>)  [unwired: 1 in]
  n17 = property on="Open" class="MCListbox (strict)"("ActiveCell"=T15 {"Row"=-2, "Column"=1} ("Active Cell:Active Cell"), "Justify"=w12, "ActiveCell"=T15 {"Row"=-2, "Column"=2} ("Active Cell:Active Cell"), "Justify"=w12) -> (error out=w13:errorcluster)  [unwired: 2 in, 1 out]
  n18 = register-events(w34) -> (reference out=w35:refnum<event-registration>)  [unwired: 2 in, 1 out]
  n19 = local write "Overrides"(T8 [{"Count"="", "Angular Override"=0.0, "Enabled?"=FALSE, "Velocity Override"=0.0, "Angle Override"=0.0}] ("Overrides")) -> ()
  n20 = call "Add First Point.vi"("Accel (f/s^2)"=w37, "Time (s)"=1 ("th"), "Initial Points"=w41) -> ("Points"=w32:cluster{"x":dbl, "y":dbl, "th":dbl}[])  [unwired: 8 in]
  n21 = local write "Tab Control"(w3) -> ()
  n22 = Bundle("Drag Object"=w29, "Hover Object"=w30, "Filename"="") -> (w28:T18)  [unwired: 1 in]
  n23 = local write "New Page Selector"(w3) -> ()
  n24 = property class="Pane"(reference=w25, "Origin"=w22) -> (error out=w21:errorcluster)  [unwired: 1 in, 1 out]
  n25 = control-ref of="Picture"() -> (w43:refnum<vi>)
  n26 = Bundle("Trajectory Data"=T12 [], "Points"=w32, "output cluster"=T14 {"Sample Period (s)"=0.2, "Limits"={"Velocity (fps)"=6.0, "Accel (fps^2)"=32.0, "Jerk (fps^3)"=1500.0, "StoopidFast (fps)"=12.0}, "Conditions"={"vInitial (fps)"=0.0, "vFinal (fps)"=0.0}, "Overrides"=[], "Angular Limits"={"Velocity (deg/s)"=0.0, "Accel (deg/s^2)"=0.0, "Jerk (deg/s^3)"=0.0}}, w19) -> (w6:T19)  [unwired: 1 in]
  n27 = while {
    tunnel: w32 -> [w117]
    tunnel: w43 -> [w116]
    shift-right: [w89] -> _
    shift-left: 0 -> [w110]
    shift-right: [w59] -> _
    shift-left: _ -> [w109]
    tunnel: w9 -> [w96]
    tunnel: w35 -> [w104]
    tunnel: w34 -> [w103]
    shift-right: [w101] -> _
    shift-left: _ -> [w102]
    shift-right: [w54] -> _
    shift-left: w6 -> [w74]
    shift-right: [w93] -> _
    shift-left: w28 -> [w94]
    shift-right: [w86] -> _
    shift-left: _ -> [w85]
    shift-right: [w83] -> _
    shift-left: "Cache" -> [w84]
    shift-right: [w76] -> _
    shift-left: w19 -> [w81]
    tunnel: w21 -> [_]
    tunnel: cluster{"width":dbl, "height":dbl}[] [{"width"=26.4166, "height"=57.5729}, {"width"=27.0, "height"=54.0}, {"width"=27.0, "height"=35.0}, {"width"=15.0, "height"=30.0}, {"width"=15.0, "height"=30.0}, {"width"=15.0, "height"=30.0}, {"width"=15.0, "height"=30.0}] -> [w71]
    tunnel: [w68] -> _
    tunnel: w13 -> [_]
    tunnel: w10 -> [w62]
    tunnel: w8 -> [w61]
    tunnel: 24.79166666666667 ("Starting Line Y") -> [w46]
    i -> [w68]
    stop <- FALSE stop-if-true
    # "False value updates pts to fit rules"
    # "tree\nupdate"
    # "New Pts"
    # "Orig Pts"
    # "Correctly sizes override array"
    # "TODO Length from vertex to blends is off because point moved.\nExtra Arc only works when enter line is at 0deg."
    # "TODO enforce points on field"
    n28 = feedback #1(w96) -> (w97:path)
    n29 = event shown="[1] \"Push\": Value Change" {
      selector: w104 -> [_ _ _ _ _ _ _ _ _ _ _ _ _ _ _ _ _ _ _ _ _ _ _ _ _ _ _]
      dyn-events: _ -> [_ _ _ _ _ _ _ _ _ _ _ _ _ _ _ _ _ _ _ _ _ _ _ _ _ _ _]
      timeout: w110 -> [_ _ _ _ _ _ _ _ _ _ _ _ _ _ _ _ _ _ _ _ _ _ _ _ _ _ _]
      tunnel: [w157 w196 w229 w269 w288 w314 w355 w370 w382 w398 w453 w485 w598 w632 w717 w744 w770 w786 w808 w827 w868 w917 w951 w1000 w1027 w1059 w1090] -> w108
      tunnel: w117 -> [_ _ w229 _ _ _ _ _ w382 w399 _ _ _ _ _ _ _ _ _ _ _ _ _ _ _ _ _]
      tunnel: w116 -> [_ _ _ _ _ _ _ _ _ _ _ w484 w584 _ w704 _ _ _ _ _ _ _ _ _ _ _ _]
      tunnel: w97 -> [w155 w194 w237 w258 w293 w311 w347 w366 w379 w403 w452 w482 w595 w650 w718 w758 w773 w788 w814 w831 w872 w923 w956 w1004 w1032 w1064 w1095]
      tunnel: [w157 w196 w234 w269 w288 w314 w355 w370 w380 w401 w453 w479 w592 w636 w702 w744 w770 w786 w808 w827 w868 w917 w951 w1000 w1027 w1059 w1090] -> w107
      tunnel: w109 -> [_ _ _ _ _ w305 _ _ _ _ _ _ _ _ _ _ _ _ _ _ _ _ _ _ _ _ _]
      tunnel: [_ _ w228 TRUE ("Flip Over Center") _ _ _ _ _ TRUE ("Flip Over Center") _ _ _ TRUE ("Flip Over Center") _ _ _ _ _ _ _ _ _ _ _ _ _] -> w60
      tunnel: [w155 w194 w237 w258 w293 w311 w347 w359 w379 w403 w452 w482 w595 w650 w718 w758 w773 w788 w814 w831 w872 w923 w956 w1004 w1032 w1064 w1095] -> w98
      tunnel: w103 -> [_ _ _ _ w292 _ _ _ _ _ _ _ _ _ _ w739 _ _ _ _ _ _ _ _ _ _ _]
      tunnel: [w159 w201 w236 w259 w291 w323 w357 w372 w387 w408 w460 w481 w594 w649 w705 w756 w772 w789 w813 w830 w871 w922 w955 w1003 w1031 w1063 w1094] -> w101
      tunnel: w102 -> [w159 w201 w236 w259 w291 _ w357 w372 w387 w408 _ w481 w594 w649 w705 w756 w772 w789 w813 w830 w871 w922 w955 w1003 w1031 w1063 w1094]
      tunnel: w74 -> [w158 w197 w235 w257 w289 w322 w356 w371 w381 w402 _ w480 w593 w648 w703 w745 w771 w787 _ w828 w869 w919 w952 w1001 w1028 w1060 w1091]
      tunnel: w94 -> [w156 w200 w233 w256 w287 w321 w352 w373 w386 w407 w468 w476 w585 w647 w700 w743 w769 w785 w812 w826 w867 w921 w954 w986 w1030 w1062 w1093]
      tunnel: [w156 w200 w233 w256 w287 w321 w353 w373 w386 w407 w468 w478 w589 w647 w700 w743 w769 w785 w812 w826 w867 w921 w954 w987 w1030 w1062 w1093] -> w93
      tunnel: [_ _ _ _ _ TRUE _ TRUE _ _ _ _ _ _ _ _ _ _ _ _ _ _ _ _ _ _ _] -> w88
      tunnel: [w154 w195 w231 w255 w286 w319 w346 w364 w385 w406 w467 w472 w587 w646 w698 w742 w764 w782 w811 w829 w870 w920 w953 w1002 w1029 w1061 w1092] -> w86
      tunnel: w85 -> [w154 w195 w231 w255 w286 w319 w346 w364 w385 w406 w467 w472 w587 w646 w698 w742 w767 w782 w811 w829 w870 w920 w953 w1002 w1029 w1061 w1092]
      tunnel: w84 -> [w153 w199 w232 w254 w285 w318 w345 w363 w384 w405 w466 w474 w586 w645 w697 w741 w766 _ w810 w815 w860 w910 w936 w984 w1013 w1050 w1078]
      tunnel: [w153 w199 w232 w254 w285 w318 w345 w363 w384 w405 w466 w474 w586 w645 w697 w741 w766 w784 w810 w815 w860 w910 w936 w984 w1013 w1050 w1078] -> w83
      tunnel: 35 -> [_ _ _ _ _ _ _ _ _ _ _ _ _ _ _ _ _ _ _ _ _ _ _ _ _ w1052 w1086]
      tunnel: w81 -> [w152 w198 _ w253 w284 w299 w354 w361 w383 w400 _ w473 w583 w644 w696 w740 w765 w783 w809 w816 w858 w915 w939 w989 w1016 w1051 w1080]
      tunnel: [w152 w198 _ w253 w284 w299 w354 w361 w383 w400 w464 w473 w583 w644 w696 w740 w765 w783 w809 w816 w862 w916 w937 w989 w1011 w1051 w1077] -> w80
      tunnel: [w151 _ w228 TRUE ("First Call?: T/F") _ _ _ _ _ TRUE ("First Call?: T/F") TRUE _ _ _ _ _ _ _ _ w819 w861 TRUE w938 _ w1015 _ TRUE] -> w79
      tunnel: w71 -> [w139 _ _ _ _ _ _ _ _ _ _ _ _ w631 _ _ _ _ _ _ _ _ _ _ _ _ _]
      tunnel: w62 -> [_ _ _ _ _ _ _ w360 _ _ _ _ _ _ _ _ _ _ _ _ _ _ _ _ _ _ _]
      tunnel: w61 -> [_ _ _ _ _ _ _ w358 _ _ _ _ _ _ _ _ _ _ _ _ _ _ _ _ _ _ _]
      tunnel: w46 -> [_ _ _ _ _ _ _ _ _ _ _ _ w576 _ w692 _ _ _ _ _ _ _ _ _ _ _ _]
      event Timeout; "Background", "Robot Color", "Robot Size (in)": Value Change {
        # "Occasionally update the listbox with all files in\nthe folder.\nAlso update the size of the picture, which field button\nis shown, color of the robot arrow,"
        n30 = event-data() -> ()  [unwired: 1 in, 1 out]
        n31 = Unbundle(w158) -> ("Updated Waypoints"=w157:cluster{"x":dbl, "y":dbl, "th":dbl}[])  [unwired: 3 out]
        n32 = call <vilib>:"Recursive File List.vi"("pattern"="*.bdx", "Folder Path"=w155) -> ("error out"=w160:errorcluster, "All Files in Dir"=w162:path[])  [unwired: 5 in, 3 out]
        n33 = Divide(x="Robot Size (in)", y=24.0 ("width")) -> (x/y=w147:cluster{"width":dbl, "height":dbl})
        n34 = for {
          tunnel: w162 -> [w169] mode=indexing
          tunnel: [w171] -> w161 mode=indexing
          tunnel: w160 -> [_]
          w163 = "%.3f" ("format string")
          n35 = call "Versioned Load.vi"("path"=w169) -> ("Overall"=w168:cluster{"Time (s)":dbl, "Distance (ft)":dbl})  [unwired: 3 in, 7 out]
          n36 = Strip Path(path=w169) -> (name=w170:string)  [unwired: 1 out]
          n37 = Unbundle(w168) -> ("Time (s)"=w167:dbl, "Distance (ft)"=w166:dbl)
          n38 = Format Into String(format string=w163, w167) -> (resulting string=w165:string)  [unwired: 2 in, 1 out]
          n39 = Format Into String(format string=w163, w166) -> (resulting string=w164:string)  [unwired: 2 in, 1 out]
          n40 = Build Array(w170, w165, w164) -> (w171:string[])
        }
        n41 = Negate(x=w147) -> (-x=w148:cluster{"width":dbl, "height":dbl})
        n42 = Unbundle(w148) -> ("width"=w146:dbl, "height"=w145:dbl)
        n43 = Unbundle(w147) -> ("width"=w144:dbl, "height"=w143:dbl)
        n44 = Index Array(array=w139, index="Background") -> (element=w138:cluster{"width":dbl, "height":dbl})
        "Field Size (ft)" <- w138
        n45 = Bundle("width"=w146, "height"=w145, "width"=w144, "height"=w143) -> (w142:T23)  [unwired: 1 in]
        n46 = global write "Global Settings.vi" "Field Size"(w138) -> ()
        n47 = global write "Global Settings.vi" "Robot Rect"(w142) -> ()
        n48 = property on="Open" class="MCListbox (strict)"("ItemNames"=w161) -> ()  [unwired: 2 in, 2 out]
        n49 = global write "Global Settings.vi" "Arrow Color"("Robot Color") -> ()
        n50 = First Call?() -> (First Call?: T/F=w151:bool)
        "RS" <- TRUE
      }
      event "Push": Value Change {
        # "Times out after\n5s"
        n51 = event-data() -> ()  [unwired: 1 in, 6 out]
        n52 = call <vilib>:"Set Busy.vi"() -> ("error out"=w173:errorcluster)  [unwired: 10 in, 1 out]
        n53 = local read "Open"() -> (w189:i32[])
        n54 = property on="Open" class="MCListbox (strict)"(error in=w173) -> ("ItemNames"=w188:string[][])  [unwired: 1 in, 2 out]
        n55 = Array Size(array=w189) -> (size(s)=w190:i32)
        n56 = Index Array(array=w189) -> (element=w191:i32)  [unwired: 1 in]
        n57 = Unbundle(w197) -> ("Updated Waypoints"=w196:cluster{"x":dbl, "y":dbl, "th":dbl}[])  [unwired: 3 out]
        n58 = Array Subset(array=w188, index (row)=w191, length (row)=w190) -> (w187:string[][])  [unwired: 2 in]
        n59 = for {
          tunnel: w187 -> [w227] mode=indexing
          tunnel: w194 -> [w221]
          tunnel: [w222] -> w186 mode=indexing
          n60 = Index Array(array=w227, index=0) -> (element=w220:string)
          n61 = Build Path(base path=w221, name or relative path=w220) -> (appended path=w219:path)
          n62 = Concatenate Strings("/home/lvuser/natinst/bin/Paths/" ("string"), w220) -> (w224:string)
          n63 = Bundle(w224, "appended path"=w219, TRUE) -> (w222:cluster{string, "appended path":path, bool})  [unwired: 1 in]
        }
        n64 = String To IP() -> (0:w180:u32)  [unwired: 1 in]
        n65 = IP To String(1:TRUE ("dot notation? (F)"), 2:w180) -> (0:w174:string)
        n66 = String Subset(string=w174, length (rest)=9 ("length (rest)")) -> (substring=w177:string)  [unwired: 1 in]
        n67 = Concatenate Strings(w177, "2" ("string")) -> (w175:string)
        n68 = call "Put Multiple Files.vi"("active (T)"=FALSE, "password"="", "user"="anonymous", "Open Connection Timeout (ms)"=5000.0, "file specifications"=w186, "host"=w175) -> ("error out"=w182:errorcluster, "file errors"=w183:errorcluster[])  [unwired: 4 in]
        n69 = Merge Errors(w183, w182) -> (w181:errorcluster)
        n70 = case shown="Error .." w181 {
          selector: w181 -> [_ w206]
          tunnel: [w202 w203] -> w172
          frame No Error {
            n71 = call "Successful"() -> ("error out"=w202:errorcluster)  [unwired: 10 in, 1 out]
          }
          frame Error {
            n72 = Equal?(x=w206, y=errorcluster {"status"=TRUE, "code"=56, "source"=""}) -> (x = y?=w210:T24)
            n73 = Unbundle By Name(w210) -> ("status"=w209:bool, "code"=w208:bool)
            n74 = Unbundle By Name(w206) -> ("code"=w204:i32, "source"=w205:string)
            n75 = And(x=w209, y=w208) -> (x .and. y?=w207:bool)
            n76 = case shown="True" w207 {
              tunnel: w205 -> [w216 _]
              tunnel: w204 -> [w215 _]
              tunnel: [w212 w218] -> w203
              frame False {
                n77 = Number To Decimal String(number=w215) -> (decimal integer string=w214:string)  [unwired: 1 in]
                n78 = Concatenate Strings("Error pushing the paths. Please see below for details:\n" ("string"), w216, w214) -> (w213:string)
                n79 = call "Error"("Message"=w213) -> ("error out"=w212:errorcluster)  [unwired: 9 in, 1 out]
              }
              frame True {
                n80 = call "Error"() -> ("error out"=w218:errorcluster)  [unwired: 10 in, 1 out]
              }
            }
          }
        }
        n81 = call <vilib>:"Unset Busy.vi"("error in (no error)"=w172) -> ()  [unwired: 10 in, 1 out]
      }
      event "New": Value Change {
        w228 = TRUE
        # "Button was pushed. Create a new trajectory path"
        # "Use Initial Location"
        n82 = event-data() -> ()  [unwired: 1 in, 5 out]
        n83 = Unbundle(w235) -> ("Updated Waypoints"=w234:cluster{"x":dbl, "y":dbl, "th":dbl}[])  [unwired: 3 out]
        n84 = local write "Conditions"(T10 {"vInitial (fps)"=0.0, "vFinal (fps)"=0.0} ("Conditions")) -> ()
      }
      event "Append": Value Change {
        # "Append button was pressed. Create a trajectory file that adopts the current position, heading, and start velocity"
        n85 = event-data() -> ()  [unwired: 1 in, 1 out]
        n86 = Unbundle(w257) -> ("Updated Waypoints"=w238:cluster{"x":dbl, "y":dbl, "th":dbl}[])  [unwired: 3 out]
        n87 = Array Size(array=w238) -> (size(s)=w247:i32)
        n88 = Decrement(x=w247) -> (x-1=w245:i32)
        n89 = Decrement(x=w245) -> (x-1=w246:i32)
        n90 = Index Array(array=w238, index=w245) -> (element=w250:cluster{"x":dbl, "y":dbl, "th":dbl})
        n91 = Index Array(array=w238, index=w246) -> (element=w244:cluster{"x":dbl, "y":dbl, "th":dbl})
        n92 = Unbundle(w250) -> ("x"=w243:dbl, "y"=w242:dbl, "th"=w249:dbl)
        n93 = Unbundle(w244) -> ("x"=w241:dbl, "y"=w240:dbl)  [unwired: 1 out]
        n94 = Not A Number/Path/Refnum?(number/path/refnum=w249) -> (NaN/Path/Refnum?=w248:bool)
        n95 = case shown="True" w248 {
          tunnel: w243 -> [_ w281]
          tunnel: w242 -> [_ w280]
          tunnel: w241 -> [_ w283]
          tunnel: w240 -> [_ w282]
          tunnel: [w271 w277] -> w239
          tunnel: w238 -> [w271 w279]
          frame False {
          }
          frame True {
            n96 = Subtract(x=w281, y=w283) -> (x-y=w272:dbl)
            n97 = Subtract(x=w280, y=w282) -> (x-y=w273:dbl)
            n98 = Delete From Array(array=w279) -> (array with subset deleted=w278:cluster{"x":dbl, "y":dbl, "th":dbl}[])  [unwired: 2 in, 1 out]
            n99 = Inverse Tangent (2 Input)(1:w272, 2:w273) -> (0:w276:dbl)
            n100 = expression code="(x/pi)*180.0" "radians to degrees"(w276) -> (w275:dbl)
            n101 = Bundle("x"=w281, "y"=w280, w275) -> (w274:cluster{"x":dbl, "y":dbl, dbl})  [unwired: 1 in]
            n102 = Build Array (concatenate)(w278, w274) -> (w277:cluster{"x":dbl, "y":dbl, "th":dbl}[])
          }
        }
        n103 = local read "Conditions"() -> (w266:T10)
        n104 = local read "Limits"() -> (w262:T9)
        n105 = Unbundle(w262) -> ("Velocity (fps)"=w261:dbl, "Accel (fps^2)"=w260:dbl)  [unwired: 2 out]
        n106 = Delete From Array(array=w239) -> (deleted portion=w268:cluster{"x":dbl, "y":dbl, "th":dbl})  [unwired: 2 in, 1 out]
        n107 = Divide(x=w261, y=w260) -> (x/y=w270:dbl)
        n108 = Build Array(w268) -> (w267:cluster{"x":dbl, "y":dbl, "th":dbl}[])
        n109 = Unbundle(w266) -> ("vFinal (fps)"=w265:dbl)  [unwired: 1 out]
        n110 = call "Add First Point.vi"("Accel (f/s^2)"=w260, "Time (s)"=w270, "Initial Points"=w267) -> ("Points"=w269:cluster{"x":dbl, "y":dbl, "th":dbl}[])  [unwired: 8 in]
        n111 = Bundle("vFinal (fps)"=w265, 0.0) -> (w264:cluster{"vFinal (fps)":dbl, dbl})  [unwired: 1 in]
        n112 = local write "Conditions"(w264) -> ()
      }
      event "Play": Value Change {
        # "Play button was pressed. Start playing the path by firing the event where it will self-feed."
        n113 = event-data() -> ()  [unwired: 1 in, 1 out]
        n114 = Unbundle(w289) -> ("Updated Waypoints"=w288:cluster{"x":dbl, "y":dbl, "th":dbl}[])  [unwired: 3 out]
        n115 = Tick Count (ms)() -> (millisecond timer value=w290:u32)
        n116 = Generate User Event(user event=w292, event data cluster=w290) -> ()  [unwired: 2 in, 2 out]
      }
      event "Save": Value Change {
        # "Negate timeout to immed update list of files"
        # "Save button was pressed. Save the file to the current directory.\nIf you modify the save code, be sure to update load as well."
        n117 = event-data() -> ()  [unwired: 1 in, 1 out]
        n118 = Unbundle By Name(w305) -> ("Time (s)"=w298:dbl, "Distance (ft)"=w303:dbl)
        n119 = Unbundle(w322) -> ("Trajectory Data"=w313:T12, "Updated Waypoints"=w314:cluster{"x":dbl, "y":dbl, "th":dbl}[], w312:T14)  [unwired: 1 out]
        n120 = local read "Drive Type"() -> (w308:T11)
        n121 = local read "Path Type"() -> (w307:T7)
        n122 = for {
          tunnel: w299 -> [w334] mode=indexing
          tunnel: w298 -> [w333]
          shift-right: [w329] -> w294
          shift-left: "" -> [w331]
          n123 = Unbundle(w334) -> ("Time (s)"=w327:dbl, w332:T3)  [unwired: 1 out]
          n124 = Unbundle By Name(w332) -> ("Name"=w328:string)
          n125 = Greater?(x=w327, y=w333) -> (0:w330:bool)
          n126 = case shown="True" w330 {
            tunnel: w331 -> [w335 w343]
            tunnel: [w335 w342] -> w329
            tunnel: w328 -> [_ w339]
            tunnel: w327 -> [_ w341]
            frame False {
            }
            frame True {
              n127 = Format Value(format string="%.2f", value (0)=w341) -> (output string=w337:string)  [unwired: 1 in]
              n128 = Concatenate Strings(w343, w339, " at " ("string"), w337, " seconds \n" ("string")) -> (w342:string)
            }
          }
        }
        n129 = Bundle("Drive Type"=w308, "Path Type"=w307) -> (w306:cluster{"Drive Type":T11, "Path Type":T7})  [unwired: 1 in]
        n130 = Select(t=nan, s="Zero Velocity", f=w303) -> (s? t:f=w301:dbl)
        n131 = Bundle("Time (s)"=w298, "Distance (ft)"=w301) -> (w300:cluster{"Time (s)":dbl, "Distance (ft)":dbl})  [unwired: 1 in]
        n132 = String Length(string=w294) -> (length=w296:i32)
        n133 = Bundle("Robot Backwards"="Robot Backwards", "Reverse Path"="Reverse Path") -> (w315:T25)  [unwired: 1 in]
        n134 = Not Equal To 0?(x=w296) -> (x != 0?=w295:bool)
        n135 = case shown="True" w295 {
          tunnel: w294 -> [_ w325]
          frame False {
          }
          frame True {
            n136 = Concatenate Strings("You have command(s) that will not be executed during this path.\nThese include:\n", w325) -> (w324:string)
            n137 = call "Display Message to User"("Message"=w324) -> ()  [unwired: 9 in, 2 out]
          }
        }
        n138 = Bundle(w315, "Trajectory Data"=w313, "sorted array out"=w299, w312, "Updated Waypoints"=w314, w300, "Zero Velocity"="Zero Velocity", w306) -> (w309:T26)  [unwired: 1 in]
        n139 = call "Versioned Write.vi"("Path stuff"=w309, "Filename"="Filename", "Bordeaux paths in"=w311) -> ()  [unwired: 9 in]
        n140 = Bundle("Trajectory Data"=w313, "Updated Waypoints"=w314, w312, "sorted array out"=w299) -> (w323:T27)  [unwired: 1 in]
      }
      event "Open Command": Value Change {
        # "Open Panel button was pressed. Open the subVI for the selected command"
        n141 = event-data() -> ()  [unwired: 1 in, 1 out]
        n142 = Unbundle(w356) -> ("Updated Waypoints"=w355:cluster{"x":dbl, "y":dbl, "th":dbl}[])  [unwired: 3 out]
        n143 = Unbundle(w345) -> ("Filtered Command Info Out"=w344:T2)  [unwired: 2 out]
        n144 = call "Open Command Panel.vi"("Cached Commands"=w344, "Commands"=w354, "Tag"="Command Sequence") -> ("Found"=w351:bool)  [unwired: 8 in]
        n145 = Select(t="Command Sequence", s=w351, f="") -> (s? t:f=w348:string)
        n146 = Bundle(cluster=w352, "Filename"=w348) -> (w353:T18)  [unwired: 2 in]
      }
      event "Directory": Value Change {
        # "Negate timeout to immed update list of files"
        # "Directory button was pressed. Put up a file dialog to let the user choose a new directory for loading and saving paths.\nUpdate the titlebar."
        n147 = event-data() -> ()  [unwired: 1 in, 1 out]
        n148 = Unbundle(w371) -> ("Updated Waypoints"=w370:cluster{"x":dbl, "y":dbl, "th":dbl}[])  [unwired: 3 out]
        n149 = call "File Dialog"("start path"=w366, "prompt"="Path Folder", "button label"="Select") -> ("selected path"=w365:path, "error out"=w367:errorcluster)  [unwired: 9 in, 2 out]
        n150 = Select(t=w366, s=w367, f=w365) -> (s? t:f=w359:path)
        n151 = call "Change Paths Directory.vi"("VI Refnum"=w358, "config path"=w360, "Bordeaux paths directory"=w359) -> ()  [unwired: 8 in, 1 out]
      }
      event "Delete": Value Change {
        n152 = event-data() -> ()  [unwired: 1 in, 6 out]
        n153 = Unbundle(w381) -> ("Updated Waypoints"=w380:cluster{"x":dbl, "y":dbl, "th":dbl}[])  [unwired: 3 out]
        n154 = local read "Open"() -> (w376:i32[])
        n155 = property on="Open" class="MCListbox (strict)"() -> ("ItemNames"=w378:string[][])  [unwired: 2 in, 2 out]
        n156 = Array Size(array=w376) -> (size(s)=w375:i32)
        n157 = Index Array(array=w376) -> (element=w377:i32)  [unwired: 1 in]
        n158 = Array Subset(array=w378, index (row)=w377, length (row)=w375) -> (w374:string[][])  [unwired: 2 in]
        n159 = for {
          tunnel: w374 -> [w394] mode=indexing
          tunnel: w379 -> [w395]
          n160 = Index Array(array=w394, index=0) -> (element=w388:string)
          n161 = String To Path(string=w388) -> (path=w389:path)
          n162 = Build Path(base path=w395, name or relative path=w389) -> (appended path=w392:path)
          n163 = Delete(path (use dialog)=w392, confirm (F)=FALSE) -> (error out=w390:errorcluster)  [unwired: 3 in, 2 out]
          n164 = call <vilib>:"Clear Errors.vi"("error in (no error)"=w390) -> ()  [unwired: 5 in, 2 out]
        }
      }
      event "Open": Shortcut Menu Selection (User) {
        n165 = event-data() -> ("ItemTag"=w404:string)  [unwired: 1 in, 7 out]
        n166 = case shown="\"False\", Default" w404 {
          tunnel: w403 -> [_ _ w421 _]
          tunnel: w402 -> [w411 w414 w418 w434]
          tunnel: [w410 w413 w417 w433] -> w401
          tunnel: w399 -> [w409 w412 w416 _]
          tunnel: [w409 w412 w416 w433] -> w398
          frame "False", Default {
            n167 = Unbundle(w411) -> ("Updated Waypoints"=w410:cluster{"x":dbl, "y":dbl, "th":dbl}[])  [unwired: 3 out]
          }
          frame "New Path" {
            n168 = Unbundle(w414) -> ("Updated Waypoints"=w413:cluster{"x":dbl, "y":dbl, "th":dbl}[])  [unwired: 3 out]
            n169 = local write "Conditions"(T10 {"vInitial (fps)"=0.0, "vFinal (fps)"=0.0} ("Conditions")) -> ()
          }
          frame "Delete Path(s)" {
            n170 = local read "Open"() -> (w419:i32[])
            n171 = Unbundle(w418) -> ("Updated Waypoints"=w417:cluster{"x":dbl, "y":dbl, "th":dbl}[])  [unwired: 3 out]
            n172 = property on="Open" class="MCListbox (strict)"() -> ("ItemNames"=w420:string[][])  [unwired: 2 in, 2 out]
            n173 = Array Size(array=w419) -> (size(s)=w423:i32)
            n174 = Index Array(array=w419) -> (element=w424:i32)  [unwired: 1 in]
            n175 = Array Subset(array=w420, index (row)=w424, length (row)=w423) -> (w422:string[][])  [unwired: 2 in]
            n176 = for {
              tunnel: w422 -> [w431] mode=indexing
              tunnel: w421 -> [w432]
              n177 = Index Array(array=w431, index=0) -> (element=w425:string)
              n178 = String To Path(string=w425) -> (path=w426:path)
              n179 = Build Path(base path=w432, name or relative path=w426) -> (appended path=w429:path)
              n180 = Delete(path (use dialog)=w429, confirm (F)=FALSE) -> (error out=w427:errorcluster)  [unwired: 3 in, 2 out]
              n181 = call <vilib>:"Clear Errors.vi"("error in (no error)"=w427) -> ()  [unwired: 5 in, 2 out]
            }
          }
          frame "Append to Path" {
            n182 = local read "Limits"() -> (w443:T9)
            n183 = Unbundle(w434) -> ("Updated Waypoints"=w436:cluster{"x":dbl, "y":dbl, "th":dbl}[])  [unwired: 3 out]
            n184 = local read "Conditions"() -> (w444:T10)
            n185 = Unbundle(w443) -> ("Velocity (fps)"=w438:dbl, "Accel (fps^2)"=w437:dbl)  [unwired: 2 out]
            n186 = Delete From Array(array=w436) -> (deleted portion=w441:cluster{"x":dbl, "y":dbl, "th":dbl})  [unwired: 2 in, 1 out]
            n187 = Divide(x=w438, y=w437) -> (x/y=w442:dbl)
            n188 = Build Array(w441) -> (w440:cluster{"x":dbl, "y":dbl, "th":dbl}[])
            n189 = Unbundle(w444) -> ("vFinal (fps)"=w439:dbl)  [unwired: 1 out]
            n190 = call "Add First Point.vi"("Accel (f/s^2)"=w437, "Time (s)"=w442, "Initial Points"=w440) -> ("Points"=w433:cluster{"x":dbl, "y":dbl, "th":dbl}[])  [unwired: 8 in]
            n191 = Bundle("vFinal (fps)"=w439, 0.0) -> (w445:cluster{"vFinal (fps)":dbl, dbl})  [unwired: 1 in]
            n192 = local write "Conditions"(w445) -> ()
          }
        }
      }
      event "Open": Double Click {
        # "When a path file is double clicked, load it and update the controls/indicators on the panel"
        n193 = event-data() -> ("Row"=w446:i32)  [unwired: 1 in, 8 out]
        n194 = property on="Open" class="MCListbox (strict)"() -> ("ItemNames"=w471:string[][])  [unwired: 2 in, 2 out]
        n195 = Index Array(array=w471, index (row)=w446, index (col)=0) -> (element=w447:string)
        n196 = Build Path(base path=w452, name or relative path=w447) -> (appended path=w470:path)
        n197 = local write "Filename"(w447) -> ()
        n198 = call "Versioned Load.vi"("path"=w470) -> ("Reversals"=w463:T25, "Trajectory Data"=w469:T12, "Zero V"=w459:bool, "Commands out"=w464:cluster{"Time (s)":dbl, T3, bool}[], "Fields"=w458:T28, "Points out"=w453:cluster{"x":dbl, "y":dbl, "th":dbl}[], "Trajectory Meta"=w451:cluster{"Drive Type":T11, "Path Type":T7})  [unwired: 3 in, 1 out]
        n199 = Unbundle(w463) -> ("Robot Backwards"=w462:bool, "Reverse Path"=w461:bool)
        n200 = Unbundle(w458) -> ("Sample Period (s)"=w457:dbl, w456:T29, "Conditions"=w455:T10, "Overrides"=w454:T8)  [unwired: 1 out]
        n201 = Unbundle(w451) -> ("Drive Type"=w450:T11, "Path Type"=w449:T7)
        n202 = local write "Robot Backwards"(w462) -> ()
        n203 = local write "Zero Velocity"(w459) -> ()
        n204 = local write "Reverse Path"(w461) -> ()
        n205 = local write "Limits"(w456) -> ()
        n206 = local write "Drive Type"(w450) -> ()
        n207 = local write "Path Type"(w449) -> ()
        n208 = local write "Sample Period (s)"(w457) -> ()
        n209 = local write "Overrides"(w454) -> ()
        n210 = local write "Conditions"(w455) -> ()
        n211 = Bundle("Trajectory Data"=w469, "Points out"=w453, "Fields"=w458, "Commands out"=w464) -> (w460:T30)  [unwired: 1 in]
      }
      event "Picture": Mouse Down {
        # "Object being clicked"
        # "Process a mouse down on the picture control. Only left clicks do anything.\nDetermine if any object was clicked on and mark it as the drag object for \nmouse move messages."
        n212 = event-data() -> ("Coords"=w486:T31, "Button"=w488:u16, "Mods"=w487:cluster{"Double Click":bool, "Menu Key":bool}, "PlatMods"=w483:T32)  [unwired: 1 in]
        n213 = Unbundle(w476) -> ("Drag Object"=w475:cluster{"Index":i32, "x":dbl, "y":dbl})  [unwired: 2 out]
        n214 = Unbundle(w480) -> ("Updated Waypoints"=w479:cluster{"x":dbl, "y":dbl, "th":dbl}[])  [unwired: 3 out]
        n215 = case shown="1" w488 {
          tunnel: w487 -> [_ _ w500]
          tunnel: w486 -> [_ _ w505]
          tunnel: w479 -> [w492 w496 w506]
          tunnel: [w492 w496 w510] -> w485
          tunnel: w484 -> [_ _ w507]
          tunnel: w475 -> [w490 w493 w501]
          tunnel: [w489 w495 w502] -> w477
          tunnel: w483 -> [_ _ w498]
          frame 0, Default {
            # "middle mouse?"
            n216 = Bundle(cluster=w490, "Index"=-1) -> (w489:cluster{"Index":i32, "x":dbl, "y":dbl})  [unwired: 2 in]
          }
          frame 2 {
            # "Right Button"
            n217 = Bundle(cluster=w493, "Index"=-1) -> (w495:cluster{"Index":i32, "x":dbl, "y":dbl})  [unwired: 2 in]
          }
          frame 1 {
            # "Left Button"
            n218 = Unbundle By Name(w500) -> ("Double Click"=w499:bool)
            n219 = property on="Picture" class="Pict"() -> ("Position"=w509:T16, "Draw Area Size"=w508:T33)  [unwired: 2 in, 2 out]
            n220 = Unbundle By Name(w498) -> ("Shift"=w497:bool)
            n221 = call "Point Test Shapes.vi"("Coords"=w505, "Points"=w506, "Picture in"=w507) -> ("Pt Test Results"=w504:enum16{"Miss", "Rect Hit", "Arrow Hit"}, "Results"=w503:T17)  [unwired: 7 in]
            n222 = case shown="\"Rect Hit\"" w504 {
              tunnel: w499 -> [_ _ w557]
              tunnel: w506 -> [w514 w542 w551]
              tunnel: w503 -> [_ w540 w558]
              tunnel: [w517 w543 w552] -> w510
              tunnel: w505 -> [w518 _ _]
              tunnel: w509 -> [w516 _ _]
              tunnel: w508 -> [w515 _ _]
              tunnel: [w512 w535 w554] -> w502
              tunnel: w501 -> [w511 _ w555]
              tunnel: w497 -> [w513 _ w547]
              frame "Miss", Default {
                n223 = case shown="True" w513 {
                  tunnel: w518 -> [w530 _]
                  tunnel: [w527 w534] -> w517
                  tunnel: w516 -> [w526 _]
                  tunnel: w515 -> [w525 _]
                  tunnel: w514 -> [w521 w534]
                  tunnel: [w520 w533] -> w512
                  tunnel: w511 -> [_ w531]
                  frame False {
                    n224 = call "Map to Feet.vi"("Draw Area Size"=w525, "Position"=w526, "Coords (px)"=w530) -> ("Point (ft)"=w524:cluster{dbl, dbl})  [unwired: 8 in]
                    n225 = Array Size(array=w521) -> (size(s)=w519:i32)
                    n226 = Unbundle(w524) -> (w523:dbl, w522:dbl)
                    n227 = Bundle(w523, w522, nan) -> (w528:cluster{dbl, dbl, dbl})  [unwired: 1 in]
                    n228 = Bundle(w519, w523, w522) -> (w520:cluster{i32, dbl, dbl})  [unwired: 1 in]
                    n229 = Build Array (concatenate)(w521, w528) -> (w527:cluster{"x":dbl, "y":dbl, "th":dbl}[])
                  }
                  frame True {
                    n230 = Bundle(cluster=w531, "Index"=-1) -> (w533:cluster{"Index":i32, "x":dbl, "y":dbl})  [unwired: 2 in]
                  }
                }
              }
              frame "Arrow Hit" {
                # "start tracking rotation"
                n231 = Unbundle(w540) -> ("Index"=w539:i32)  [unwired: 1 out]
                n232 = Index Array(array=w542, index=w539) -> (element=w541:cluster{"x":dbl, "y":dbl, "th":dbl})
                n233 = Unbundle(w541) -> ("x"=w538:dbl, "y"=w537:dbl, "th"=w545:dbl)
                n234 = Bundle(cluster=w541, "th"=w545) -> (w544:cluster{"x":dbl, "y":dbl, "th":dbl})  [unwired: 2 in]
                n235 = Bundle(-2, "x"=w538, "y"=w537) -> (w535:cluster{i32, "x":dbl, "y":dbl})  [unwired: 1 in]
                n236 = Replace Array Subset(array=w542, new element=w544) -> (w543:cluster{"x":dbl, "y":dbl, "th":dbl}[])  [unwired: 1 in]
              }
              frame "Rect Hit" {
                n237 = Unbundle(w558) -> ("Index"=w556:i32)  [unwired: 1 out]
                n238 = Array Size(array=w551) -> (size(s)=w550:i32)
                n239 = Greater?(x=w550, y=2) -> (0:w548:bool)
                n240 = And(x=w547, y=w548) -> (x .and. y?=w546:bool)
                n241 = case shown="True" w546 {
                  tunnel: w557 -> [w562 _]
                  tunnel: w556 -> [w561 w565]
                  tunnel: [w560 -1 ("length")] -> w553
                  tunnel: w551 -> [w559 w568]
                  tunnel: [w559 w567] -> w552
                  frame False {
                    n242 = case shown="False" w562 {
                      tunnel: w561 -> [w563 _]
                      tunnel: [w563 -1] -> w560
                      frame False {
                      }
                      frame True {
                        # "TODO Toggle last pt"
                      }
                    }
                  }
                  frame True {
                    n243 = case shown="0" w565 {
                      tunnel: w568 -> [w569 w573]
                      tunnel: w565 -> [_ w572]
                      tunnel: [w569 w570] -> w567
                      frame 0 {
                      }
                      frame Default {
                        n244 = Delete From Array(array=w573, length=1, index=w572) -> (array with subset deleted=w570:cluster{"x":dbl, "y":dbl, "th":dbl}[])  [unwired: 1 out]
                      }
                    }
                  }
                }
                n245 = Bundle(cluster=w555, "Index"=w553) -> (w554:cluster{"Index":i32, "x":dbl, "y":dbl})  [unwired: 2 in]
              }
            }
          }
        }
        n246 = Bundle(cluster=w476, "Drag Object"=w477) -> (w478:T18)  [unwired: 2 in]
      }
      event "Picture": Mouse Move; "Picture": Mouse Up {
        # "If an object was clicked on and is being moved, update position.\nIf nothing is being dragged, you may be hovering over an object and\nwant to draw it differently."
        n247 = event-data() -> ("Type"=w597:T21, "Coords"=w599:T31)  [unwired: 1 in]
        n248 = local read "Robot Size (in)"() -> (w579:cluster{"width":dbl, "height":dbl})
        n249 = Unbundle By Name(w579) -> ("width"=w577:dbl)
        n250 = Divide(x=w577, y=24.0) -> (x/y=w575:dbl)
        n251 = Subtract(x=w576, y=w575) -> (x-y=w574:dbl)
        n252 = Unbundle(w593) -> ("Updated Waypoints"=w592:cluster{"x":dbl, "y":dbl, "th":dbl}[])  [unwired: 3 out]
        n253 = Unbundle(w585) -> ("Drag Object"=w588:cluster{"Index":i32, "x":dbl, "y":dbl})  [unwired: 2 out]
        n254 = Unbundle(w588) -> ("Index"=w596:i32)  [unwired: 2 out]
        n255 = case shown="Default" w596 {
          selector: w596 -> [w610 _]
          tunnel: w599 -> [w619 w627]
          tunnel: [w617 w626] -> w590
          tunnel: [w614 w625] -> w598
          tunnel: w592 -> [w615 w625]
          tunnel: [w611 w624] -> w591
          tunnel: w588 -> [w602 w624]
          tunnel: w597 -> [w612 _]
          tunnel: "Snap to foot" -> [w607 _]
          tunnel: "Snap robot to baseline" -> [w608 _]
          tunnel: "Angle Limiter" -> [w609 _]
          tunnel: w584 -> [w601 w623]
          tunnel: w583 -> [_ w622]
          tunnel: w574 -> [w600 _]
          frame Default {
            # "Mouse up changes indes to break tracking,\notherwise update coords"
            n256 = property on="Picture" class="Pict"() -> ("Position"=w620:T16, "Draw Area Size"=w621:T33)  [unwired: 2 in, 2 out]
            n257 = Bundle("Snap robot to baseline"=w608, "Snap to foot"=w607, "Angle Limiter"=w609) -> (w606:T34)  [unwired: 1 in]
            n258 = Equal?(x=lveventtype."Mouse Up" ("Type"), y=w612) -> (x = y?=w605:bool)
            n259 = call "Map to Feet.vi"("Draw Area Size"=w621, "Position"=w620, "Coords (px)"=w619) -> ("Point (ft)"=w618:cluster{dbl, dbl})  [unwired: 8 in]
            n260 = call "Handle Pos and Rot.vi"("Starting Line Y"=w600, "Mouse Up"=w605, "Picture in"=w601, "Option"=w606, "Coord (ft)"=w618, "Index"=w610, "Points in"=w615) -> ("Points out"=w614:cluster{"x":dbl, "y":dbl, "th":dbl}[])  [unwired: 4 in]
            n261 = Bundle(cluster=w602, "Index"=-1) -> (w603:cluster{"Index":i32, "x":dbl, "y":dbl})  [unwired: 2 in]
            n262 = Bundle(w610, "Pt Test Results"=enum16{"Miss", "Rect Hit", "Arrow Hit"}."Rect Hit") -> (w617:T35)  [unwired: 1 in]
            n263 = Select(t=w603, s=w605, f=w602) -> (s? t:f=w611:cluster{"Index":i32, "x":dbl, "y":dbl})
          }
          frame -1 {
            n264 = call "Point Test Shapes.vi"("Array"=w622, "Coords"=w627, "Points"=w625, "Picture in"=w623) -> ("Results"=w626:T17)  [unwired: 6 in, 1 out]
          }
        }
        n265 = Bundle(cluster=w585, "Drag Object"=w591, "Hover Object"=w590) -> (w589:T18)  [unwired: 1 in]
      }
      event "Time (s)", "Sample Period (s)", "Horizontal Reflection", "Conditions", "Vertical Reflection": Value Change {
        # "Don't updates pts to fit rules"
        # "Changes to any of these controls will update the picture and other indicators to be consistent."
        n266 = event-data() -> ("CtlRef"=w639:refnum<vi>)  [unwired: 1 in]
        n267 = control-ref of="Vertical Reflection"() -> (w638:refnum<vi>)
        n268 = control-ref of="Horizontal Reflection"() -> (w652:refnum<vi>)
        n269 = Index Array(array=w631) -> (element=w630:cluster{"width":dbl, "height":dbl})  [unwired: 1 in]
        n270 = Unbundle By Name(w630) -> ("width"=w629:dbl, "height"=w628:dbl)
        n271 = Equal?(x=w652, y=w639) -> (x = y?=w633:bool)
        n272 = Equal?(x=w639, y=w638) -> (x = y?=w637:bool)
        n273 = Unbundle(w648) -> ("Updated Waypoints"=w636:cluster{"x":dbl, "y":dbl, "th":dbl}[])  [unwired: 3 out]
        n274 = case shown="True" w633 {
          tunnel: w636 -> [w668 w671]
          tunnel: [w668 w670] -> w635
          tunnel: w629 -> [_ w669]
          frame False {
          }
          frame True {
            n275 = for {
              tunnel: w671 -> [w681] mode=indexing
              tunnel: [w678] -> w670 mode=indexing
              tunnel: w669 -> [w675]
              n276 = Unbundle(w681) -> ("x"=w680:dbl, "y"=w679:dbl, "th"=w673:dbl)
              n277 = Negate(x=w680) -> (-x=w677:dbl)
              n278 = Subtract(x=180.0, y=w673) -> (x-y=w672:dbl)
              n279 = Add(x=w675, y=w677) -> (x+y=w676:dbl)
              n280 = Bundle(w676, "y"=w679, w672) -> (w678:cluster{dbl, "y":dbl, dbl})  [unwired: 1 in]
            }
          }
        }
        n281 = case shown="True" w637 {
          tunnel: w636 -> [w653 w656]
          tunnel: [w653 w655] -> w634
          tunnel: w628 -> [_ w654]
          frame False {
          }
          frame True {
            n282 = for {
              tunnel: w656 -> [w666] mode=indexing
              tunnel: [w667] -> w655 mode=indexing
              tunnel: w654 -> [w657]
              n283 = Unbundle By Name(w666) -> ("y"=w665:dbl, "x"=w664:dbl, "th"=w661:dbl)
              n284 = Negate(x=w665) -> (-x=w659:dbl)
              n285 = Negate(x=w661) -> (-x=w660:dbl)
              n286 = Add(x=w657, y=w659) -> (x+y=w658:dbl)
              n287 = Swap Values(12:w658, 14:w664) -> (1:w663:dbl, 3:w662:dbl)  [unwired: 1 in]
              n288 = Bundle(w663, w662, w660) -> (w667:cluster{dbl, dbl, dbl})  [unwired: 1 in]
            }
          }
        }
        n289 = Select(t=w635, s=w633, f=w634) -> (s? t:f=w632:cluster{"x":dbl, "y":dbl, "th":dbl}[])
        n290 = local read "Path Type"() -> (w643:T7)
        n291 = case shown="\"Clothoid\", Default" w643 {
          tunnel: "Unjank" -> [_ w685]
          tunnel: w648 -> [_ w684]
          tunnel: "Turn Acceleration" -> [_ w683]
          tunnel: "Turn Deceleration" -> [_ w682]
          frame "Bezier" {
          }
          frame "Clothoid", Default {
            n292 = case shown="True" w685 {
              tunnel: w684 -> [_ w686]
              tunnel: w683 -> [_ w689]
              tunnel: w682 -> [_ w688]
              frame False {
              }
              frame True {
                n293 = call "Turn Smother.vi"("Ignore Deceleration"=w688, "Ignore Acceleration"=w689, "Internal Path Stuff"=w686) -> ("Overrides"=w687:T8)  [unwired: 1 in]
                n294 = local write "Overrides"(w687) -> ()
              }
            }
          }
        }
      }
      event Key Down?; event type 5.0.x8000000b {
        # "If hovering over an object, nudge using arrow keys"
        n295 = event-data() -> ("VKey"=w709:T36)  [unwired: 1 in]
        n296 = local read "Robot Size (in)"() -> (w691:cluster{"width":dbl, "height":dbl})
        n297 = Unbundle By Name(w691) -> ("width"=w694:dbl)
        n298 = Divide(x=w694, y=24.0) -> (x/y=w693:dbl)
        n299 = local read "Snap robot to baseline"() -> (w716:bool)
        n300 = Unbundle(w703) -> ("Updated Waypoints"=w702:cluster{"x":dbl, "y":dbl, "th":dbl}[])  [unwired: 3 out]
        n301 = Subtract(x=w692, y=w693) -> (x-y=w690:dbl)
        n302 = local read "Angle Limiter"() -> (w714:enum16{"90", "45", "15", "1"})
        n303 = local read "Snap to foot"() -> (w715:bool)
        n304 = Unbundle(w700) -> ("Hover Object"=w701:T17)  [unwired: 2 out]
        n305 = case shown="\"Up\"" w709 {
          tunnel: [cluster{dbl, dbl} {0.0, 0.0} ("Coord (ft)") cluster{dbl, dbl} {0.0, 0.1} ("Coord (ft)") cluster{dbl, dbl} {0.0, -0.1} ("Coord (ft)") cluster{dbl, dbl} {-0.1, 0.0} ("Coord (ft)") cluster{dbl, dbl} {0.1, 0.0} ("Coord (ft)")] -> w711
          tunnel: [_ w730 w732 w734 w736] -> w707
          tunnel: TRUE ("Delta") -> [_ w730 w732 w734 w736]
          frame Default {
          }
          frame "Up" {
          }
          frame "Down" {
          }
          frame "Left" {
          }
          frame "Right" {
          }
        }
        n306 = Unbundle(w701) -> ("Index"=w699:i32, "Pt Test Results"=w708:enum16{"Miss", "Rect Hit", "Arrow Hit"})
        n307 = Bundle("Snap robot to baseline"=w716, "Snap to foot"=w715, "Angle Limiter"=w714) -> (w713:T34)  [unwired: 1 in]
        n308 = case shown="\"Rect Hit\", Default" w708 {
          tunnel: [w719 w728] -> w717
          tunnel: w704 -> [_ w727]
          tunnel: w713 -> [_ w726]
          tunnel: w702 -> [w719 w725]
          tunnel: TRUE ("Delta") -> [_ w724]
          tunnel: w711 -> [_ w723]
          tunnel: w707 -> [_ w722]
          tunnel: [_ w722] -> w706
          tunnel: w699 -> [_ w721]
          tunnel: w690 -> [_ w720]
          frame "Miss" {
          }
          frame "Rect Hit", Default {
            n309 = call "Handle Pos and Rot.vi"("Starting Line Y"=w720, "Delta"=w724, "Picture in"=w727, "Option"=w726, "Coord (ft)"=w723, "Index"=w721, "Points in"=w725) -> ("Points out"=w728:cluster{"x":dbl, "y":dbl, "th":dbl}[])  [unwired: 4 in]
          }
        }
        n310 = event-data("Discard?"=w706) -> ()  [unwired: 1 in, 1 out]
      }
      event User Event {
        # "Fire events to animate the timeline\nuntil we reach the end"
        n311 = event-data() -> ("Data"=w752:i32)  [unwired: 1 in]
        n312 = Unbundle(w745) -> ("Updated Waypoints"=w744:cluster{"x":dbl, "y":dbl, "th":dbl}[])  [unwired: 3 out]
        n313 = Tick Count (ms)() -> (millisecond timer value=w755:u32)
        n314 = Subtract(x=w755, y=w752) -> (x-y=w754:u32)
        n315 = Multiply(x=w754, y=0.001) -> (x*y=w751:dbl)
        n316 = local read "Duration (s)"() -> (w738:dbl)
        n317 = Quotient & Remainder(x=w751, y=0.02) -> (floor(x/y)=w749:dbl)  [unwired: 1 out]
        n318 = Wait (ms)(milliseconds to wait=u32 50) -> ()  [unwired: 1 out]
        n319 = Multiply(x=0.02, y=w749) -> (x*y=w748:dbl)
        n320 = Less Or Equal?(x=w748, y=w738) -> (x <= y?=w757:bool)
        n321 = case shown="True" w757 {
          tunnel: w739 -> [_ w762]
          tunnel: w752 -> [_ w760]
          tunnel: w748 -> [_ w761]
          tunnel: w738 -> [w759 _]
          frame False {
            n322 = local write "Time (s)"(w759) -> ()
          }
          frame True {
            n323 = Generate User Event(user event=w762, event data cluster=w760) -> ()  [unwired: 2 in, 2 out]
            n324 = local write "Time (s)"(w761) -> ()
          }
        }
      }
      event "New Page Selector": Value Change {
        # "If looking at the commands, look at projects for one with a RIO target"
        n325 = event-data() -> ("NewVal"=w768:T1)  [unwired: 1 in]
        n326 = Unbundle(w771) -> ("Updated Waypoints"=w770:cluster{"x":dbl, "y":dbl, "th":dbl}[])  [unwired: 3 out]
        n327 = case shown="\"Command Sequencer\"" w768 {
          tunnel: [w774 w775] -> w764
          tunnel: w767 -> [w774 _]
          frame "Trajectory Settings", Default {
          }
          frame "Command Sequencer" {
            n328 = call "Find RT Projects.vi"() -> ("Paths"=w776:path[], "Targets"=w777:refnum<vi>[], "Project Names"=w778:string[])  [unwired: 9 in]
            n329 = property on="Projects" class="Ring (strict)"("Strings []"=w778) -> ()  [unwired: 2 in, 2 out]
            n330 = Bundle("Targets"=w777, "Paths"=w776) -> (w775:cluster{"Targets":refnum<vi>[], "Paths":path[]})  [unwired: 1 in]
          }
        }
        n331 = local write "Tab Control"("New Page Selector") -> ()
      }
      event "Refresh": Value Change {
        # "Refresh button was pressed. Reload the command info from the project.\nLater, maybe store this in a file because it takes awhile to recompute."
        n332 = event-data() -> ()  [unwired: 1 in, 1 out]
        n333 = Unbundle(w787) -> ("Updated Waypoints"=w786:cluster{"x":dbl, "y":dbl, "th":dbl}[])  [unwired: 3 out]
        n334 = flat-sequence {
          tunnel: [w790] -> w780
          tunnel: w782 -> [w797]
          tunnel: [w801] -> w781
          tunnel: w780 -> [w791]
          tunnel: [w791] -> w779
          tunnel: [w807] -> w784
          tunnel: w781 -> [w807]
          tunnel: w779 -> [w806]
          frame #0 {
            n335 = call <vilib>:"Set Busy.vi"() -> ("error out"=w790:errorcluster)  [unwired: 10 in, 1 out]
          }
          frame #1 {
            n336 = Unbundle(w797) -> ("Targets"=w796:refnum<vi>[], "Paths"=w795:path[])
            n337 = Index Array(array=w796, index="Projects") -> (element=w805:refnum<vi>)
            n338 = Index Array(array=w795, index="Projects") -> (element=w793:path)
            n339 = Strip Path(path=w793) -> (stripped path=w792:path)  [unwired: 1 out]
            n340 = global read "Global Settings.vi" "Icon Scale Factor"() -> (w798:dbl)
            n341 = call "Find Command Names.vi"("project root path"=w792, "TargetItem in"=w805) -> ("Paths"=w804:path[], "Command Info"=w803:T37)  [unwired: 8 in]
            n342 = call "Format Commands to Tree.vi"("Paths"=w804, "Command Info"=w803) -> ("2D Picture"=w802:picture, "Filtered Command Info Out"=w800:T2)  [unwired: 8 in]
            n343 = call "Resize Icons.vi"("Scale Factor"=w798, "Filtered Command Info Out"=w800) -> ("Filtered Command Info Out"=w799:T2)  [unwired: 9 in]
            n344 = Bundle("Filtered Command Info Out"=w799, "2D Picture"=w802, "stripped path"=w792) -> (w801:T38)  [unwired: 1 in]
            n345 = local write "Command Palette"(w802) -> ()
            n346 = local write "Cache"(w801) -> ()
          }
          frame #2 {
            n347 = call <vilib>:"Unset Busy.vi"("error in (no error)"=w806) -> ()  [unwired: 10 in, 1 out]
          }
        }
        n348 = call-poly <vilib>:"Set Cursor.vi"() -> ()  [unwired: 10 in, 2 out]
      }
      event "WayPoints": Value Change {
        # "If the waypoints control is hand-edited, pass the new data along to update the picture and other indicators\nand make it consistent"
        n349 = event-data() -> ("NewVal"=w808:cluster{"x":dbl, "y":dbl, "th":dbl}[])  [unwired: 1 in]
      }
      event event #0x53 {
        # "This is an alternative to the Inhale button. Notice that it doesn't actually modify anything at the\nmoment."
        n350 = event-data() -> ("VIName"=w818:string)  [unwired: 1 in]
        n351 = Unbundle(w828) -> ("Updated Waypoints"=w827:cluster{"x":dbl, "y":dbl, "th":dbl}[])  [unwired: 3 out]
        n352 = Unbundle(w826) -> ("Filename"=w817:string)  [unwired: 2 out]
        n353 = Search and Replace String(input string=w817, search string=w818, replace string=w818) -> (number of replacements=w823:i32)  [unwired: 5 in, 3 out]
        n354 = call "Find Command with Tag.vi"("Command Tag"=w817, "Commands"=w816) -> ("Index"=w824:i32, "Found Command"=w825:cluster{"Time (s)":dbl, T3, bool}, "Found"=w821:bool)  [unwired: 7 in]
        n355 = Not Equal To 0?(x=w823) -> (x != 0?=w822:bool)
        n356 = And(x=w821, y=w822) -> (x .and. y?=w820:bool)
        n357 = disable-structure shown="Disabled" {
          disable-tunnel: w825 -> [w836 _]
          disable-tunnel: w824 -> [w835 _]
          disable-tunnel: w820 -> [w834 _]
          disable-tunnel: [w833 _] -> w819
          disable-tunnel: w816 -> [w832 _]
          frame Disabled {
            n358 = case shown="True" w834 {
              tunnel: w836 -> [_ w843]
              tunnel: w835 -> [_ w850]
              tunnel: w832 -> [w837 w852]
              tunnel: [w837 w851] -> _
              tunnel: [_ FALSE] -> w833
              frame False {
              }
              frame True {
                n359 = Unbundle(w843) -> (w845:T3)  [unwired: 2 out]
                n360 = Unbundle(w845) -> ("Path"=w849:path)  [unwired: 6 out]
                n361 = Open VI Reference(vi path=w849) -> (vi reference=w847:refnum<vi>)  [unwired: 5 in, 1 out]
                n362 = property class="VI"(reference=w847) -> (reference out=w840:refnum<vi>, "Panel"=w848:refnum<vi>)  [unwired: 1 in, 1 out]
                n363 = property class="Pnl"(reference=w848) -> ("Controls[]"=w846:refnum<vi>[])  [unwired: 1 in, 2 out]
                n364 = for {
                  tunnel: w846 -> [w857] mode=indexing
                  tunnel: [w854] -> w844 mode=indexing
                  shift-right: [w853] -> w839
                  shift-left: w840 -> [w853]
                  n365 = property class="Ctl"(reference=w857) -> ("Label.Text"=w856:string, "Value"=w855:variant)  [unwired: 1 in, 2 out]
                  n366 = Bundle("Label.Text"=w856, "Value"=w855) -> (w854:cluster{"Label.Text":string, "Value":variant})  [unwired: 1 in]
                }
                n367 = Bundle(cluster=w845, "All Control Values Variant"=w844) -> (w842:T3)  [unwired: 6 in]
                n368 = Bundle(cluster=w843, w842) -> (w841:cluster{"Time (s)":dbl, T3, bool})  [unwired: 2 in]
                n369 = Replace Array Subset(array=w852, new element=w841, index=w850) -> (w851:cluster{"Time (s)":dbl, T3, bool}[])
                n370 = Close Reference(reference=w839) -> ()  [unwired: 1 in, 1 out]
              }
            }
          }
          frame Enabled {
          }
        }
      }
      event "Inhale": Value Change {
        # "Inhale button was pressed. Get the value of the controls/parameters and make them the\nvalues that will be used for the command."
        n371 = event-data() -> ()  [unwired: 1 in, 1 out]
        n372 = Unbundle(w869) -> ("Updated Waypoints"=w868:cluster{"x":dbl, "y":dbl, "th":dbl}[])  [unwired: 3 out]
        n373 = Unbundle(w867) -> ("Filename"=w866:string)  [unwired: 2 out]
        n374 = Unbundle(w860) -> ("Filtered Command Info Out"=w859:T2)  [unwired: 2 out]
        n375 = call "Find Command with Tag.vi"("Command Tag"=w866, "Commands"=w858) -> ("Index"=w863:i32, "Found Command"=w864:cluster{"Time (s)":dbl, T3, bool}, "Found"=w865:bool)  [unwired: 7 in]
        n376 = case shown="True" w865 {
          tunnel: w864 -> [_ w890]
          tunnel: w863 -> [_ w896]
          tunnel: w858 -> [w873 w898]
          tunnel: [w873 w897] -> w862
          tunnel: [_ TRUE] -> w861
          tunnel: w859 -> [_ w875]
          frame False {
          }
          frame True {
            n377 = Unbundle(w890) -> (w892:T3)  [unwired: 2 out]
            n378 = Unbundle(w892) -> ("Name"=w876:string, "Path"=w895:path)  [unwired: 5 out]
            n379 = Open VI Reference(vi path=w895) -> (vi reference=w877:refnum<vi>, error out=w881:errorcluster)  [unwired: 5 in]
            n380 = Unbundle(w881) -> ("code"=w880:i32)  [unwired: 2 out]
            n381 = Not Equal?(x=w880, y=0) -> (x != y?=w878:bool)
            n382 = case shown="False" w878 {
              tunnel: w877 -> [w899 w903]
              tunnel: w876 -> [_ w902]
              tunnel: w875 -> [_ w901]
              tunnel: [w899 w900] -> w874
              frame False {
              }
              frame True {
                n383 = call "Replace Command with Cached Command.vi"("Cached Commands"=w901, "Name"=w902, "VI in"=w903) -> ("VI out"=w900:refnum<vi>)  [unwired: 8 in]
              }
            }
            n384 = property class="VI"(reference=w874) -> (reference out=w887:refnum<vi>, "Panel"=w894:refnum<vi>)  [unwired: 1 in, 1 out]
            n385 = property class="Pnl"(reference=w894) -> (reference out=w885:refnum<vi>, "Controls[]"=w893:refnum<vi>[])  [unwired: 1 in, 1 out]
            n386 = for {
              tunnel: w893 -> [w909] mode=indexing
              tunnel: [w906] -> w891 mode=indexing
              shift-right: [w905] -> w884
              shift-left: w887 -> [w905]
              shift-right: [w904] -> _
              shift-left: w885 -> [w904]
              n387 = property class="Ctl"(reference=w909) -> ("Label.Text"=w908:string, "Value"=w907:variant)  [unwired: 1 in, 2 out]
              n388 = Bundle("Label.Text"=w908, "Value"=w907) -> (w906:cluster{"Label.Text":string, "Value":variant})  [unwired: 1 in]
            }
            n389 = Bundle(cluster=w892, "All Control Values Variant"=w891) -> (w889:T3)  [unwired: 6 in]
            n390 = Bundle(cluster=w890, w889) -> (w888:cluster{"Time (s)":dbl, T3, bool})  [unwired: 2 in]
            n391 = Replace Array Subset(array=w898, new element=w888, index=w896) -> (w897:cluster{"Time (s)":dbl, T3, bool}[])
            n392 = property class="VI"(reference=w884, "FP.State"=T22."Closed" ("Front Panel Window:State")) -> (reference out=w883:refnum<vi>)  [unwired: 1 in, 1 out]
            n393 = Close Reference(reference=w883) -> ()  [unwired: 1 in, 1 out]
          }
        }
      }
      event "fps": Cursor Move {
        # "The red cursor on the velocity graph was moved to a new location. Update the time slider to be in sync"
        n394 = event-data() -> ("CursIdx"=w912:i32, "CursLoc"=w918:cluster{"X":dbl, "Y":dbl})  [unwired: 1 in]
        n395 = Unbundle(w919) -> ("Updated Waypoints"=w917:cluster{"x":dbl, "y":dbl, "th":dbl}[])  [unwired: 3 out]
        n396 = Array Size(array=w915) -> (size(s)=w914:i32)
        n397 = Greater?(x=w914, y=w912) -> (0:w913:bool)
        n398 = case shown="False" w913 {
          tunnel: w918 -> [w926 w931]
          tunnel: w915 -> [w924 w929]
          tunnel: [w924 w928] -> w916
          tunnel: w912 -> [_ w927]
          frame False {
            n399 = Unbundle(w926) -> ("X"=w925:dbl)  [unwired: 1 out]
            n400 = local write "Time (s)"(w925) -> ()
          }
          frame True {
            n401 = Unbundle(w931) -> ("X"=w930:dbl)  [unwired: 1 out]
            n402 = in-place {
              in-place-border: w930 -> [w934]
              n403 = in-place-array #2(w929, w927) -> (w933:cluster{"Time (s)":dbl, T3, bool})
              n404 = Bundle(cluster=w933, "Time (s)"=w934) -> (w932:cluster{"Time (s)":dbl, T3, bool})  [unwired: 2 in]
              n405 = in-place-array #2(w932) -> (w928:cluster{"Time (s)":dbl, T3, bool}[])  [unwired: 1 out]
            }
          }
        }
      }
      event "Command Sequence": Mouse Down {
        # "second column, tag starting with // indicates an enable click"
        # "Handle a click on a row of the tree within the Command Sequencer tab.\nThis only handles the enable/disable click"
        n406 = event-data() -> ("CtlRef"=w949:refnum<vi>, "Coords"=w950:T31, "PlatMods.Shift"=w935:bool)  [unwired: 1 in]
        n407 = Unbundle(w952) -> ("Updated Waypoints"=w951:cluster{"x":dbl, "y":dbl, "th":dbl}[])  [unwired: 3 out]
        n408 = invoke class="Tree (strict)" method="Point To Row Column"(reference=w949, "Point"=w950) -> ("Tag"=w940:string, "Col"=w944:i32)  [unwired: 6 in, 6 out]
        n409 = String Subset(string=w940, length (rest)=2 ("length (rest)")) -> (substring=w948:string)  [unwired: 1 in]
        n410 = Equal?(x=2 ("length (rest)"), y=w944) -> (x = y?=w943:bool)
        n411 = Equal?(x="//", y=w948) -> (x = y?=w942:bool)
        n412 = And(x=w942, y=w943) -> (x .and. y?=w941:bool)
        n413 = case shown="True" w941 {
          tunnel: w939 -> [w957 w960]
          tunnel: w940 -> [_ w964]
          tunnel: [w957 w959] -> w937
          tunnel: [_ TRUE] -> w938
          tunnel: w935 -> [_ w958]
          frame False {
          }
          frame True {
            # "click on enable of a command"
            n414 = call "Find Command with Tag.vi"("Command Tag"=w964, "Commands"=w960) -> ("Index"=w961:i32, "Found Command"=w962:cluster{"Time (s)":dbl, T3, bool}, "Found"=w963:bool)  [unwired: 7 in]
            n415 = case shown="False" w958 {
              tunnel: w963 -> [w970 _]
              tunnel: w962 -> [w969 _]
              tunnel: w961 -> [w968 w979]
              tunnel: w960 -> [w967 w982]
              tunnel: [w966 w981] -> w959
              frame False {
                # "Toggle"
                n416 = case shown="True" w970 {
                  tunnel: w969 -> [_ w973]
                  tunnel: w968 -> [_ w976]
                  tunnel: w967 -> [w971 w977]
                  tunnel: [w971 w974] -> w966
                  frame False {
                  }
                  frame True {
                    n417 = Unbundle(w973) -> (w972:bool)  [unwired: 2 out]
                    n418 = Not(x=w972) -> (.not. x?=w978:bool)
                    n419 = Bundle(cluster=w973, w978) -> (w975:cluster{"Time (s)":dbl, T3, bool})  [unwired: 2 in]
                    n420 = Replace Array Subset(array=w977, new element=w975, index=w976) -> (w974:cluster{"Time (s)":dbl, T3, bool}[])
                  }
                }
              }
              frame True {
                # "Delete"
                n421 = Delete From Array(array=w982, length=1, index=w979) -> (array with subset deleted=w981:cluster{"Time (s)":dbl, T3, bool}[])  [unwired: 1 out]
              }
            }
          }
        }
      }
      event "Command Sequence": Double Click {
        # "This handles a double-click of a command in the first column. This opens the panel \nand updates the parameters to the values in the command."
        n422 = event-data() -> ("CtlRef"=w998:refnum<vi>, "Coords"=w999:T31)  [unwired: 1 in]
        n423 = Unbundle(w1001) -> ("Updated Waypoints"=w1000:cluster{"x":dbl, "y":dbl, "th":dbl}[])  [unwired: 3 out]
        n424 = invoke class="Tree (strict)" method="Point To Row Column"(reference=w998, "Point"=w999) -> ("Tag"=w988:string, "Col"=w993:i32)  [unwired: 6 in, 6 out]
        n425 = String Subset(string=w988, length (rest)=2 ("length (rest)")) -> (substring=w997:string)  [unwired: 1 in]
        n426 = Equal?(x=0 ("length (rest)"), y=w993) -> (x = y?=w992:bool)
        n427 = Equal?(x="//", y=w997) -> (x = y?=w991:bool)
        n428 = And(x=w991, y=w992) -> (x .and. y?=w990:bool)
        n429 = Unbundle(w984) -> ("Filtered Command Info Out"=w983:T2)  [unwired: 2 out]
        n430 = case shown="True" w990 {
          tunnel: w989 -> [_ w1010]
          tunnel: w988 -> [_ w1008]
          tunnel: [_ w1007] -> w985
          tunnel: w983 -> [_ w1005]
          frame False {
          }
          frame True {
            n431 = call "Open Command Panel.vi"("Cached Commands"=w1005, "Commands"=w1010, "Tag"=w1008) -> ("Found"=w1009:bool)  [unwired: 8 in]
            n432 = Select(t=w1008, s=w1009, f="") -> (s? t:f=w1007:string)
          }
        }
        n433 = Bundle(cluster=w986, "Filename"=w985) -> (w987:T18)  [unwired: 2 in]
      }
      event "Command Sequence": Edit Cell? {
        # "This allows you to enter time  directly using the tree cell"
        n434 = event-data() -> ("String"=w1019:string, "Tag"=w1018:string, "Col"=w1021:i32)  [unwired: 1 in]
        n435 = Unbundle(w1028) -> ("Updated Waypoints"=w1027:cluster{"x":dbl, "y":dbl, "th":dbl}[])  [unwired: 3 out]
        n436 = Equal?(x=1 ("length (rest)"), y=w1021) -> (x = y?=w1022:bool)
        n437 = String Subset(string=w1018, length (rest)=2 ("length (rest)")) -> (substring=w1026:string)  [unwired: 1 in]
        n438 = Equal?(x="//", y=w1026) -> (x = y?=w1023:bool)
        n439 = And(x=w1023, y=w1022) -> (x .and. y?=w1020:bool)
        n440 = case shown="True" w1020 {
          tunnel: [TRUE _] -> w1014
          tunnel: w1019 -> [_ w1042]
          tunnel: w1016 -> [w1033 w1039]
          tunnel: w1018 -> [_ w1038]
          tunnel: [w1033 w1040] -> w1012
          frame False {
          }
          frame True {
            n441 = call "Find Command with Tag.vi"("Command Tag"=w1038, "Commands"=w1039) -> ("Index"=w1036:i32, "Found Command"=w1035:cluster{"Time (s)":dbl, T3, bool}, "Found"=w1037:bool)  [unwired: 7 in]
            n442 = Scan From String(input string=w1042) -> (output 1=w1041:dbl)  [unwired: 4 in, 3 out]
            n443 = case shown="True" w1037 {
              tunnel: w1039 -> [w1043 w1046]
              tunnel: [w1043 w1047] -> w1040
              tunnel: w1041 -> [_ w1048]
              tunnel: w1036 -> [_ w1044]
              tunnel: w1035 -> [_ w1049]
              frame False {
              }
              frame True {
                n444 = Bundle(cluster=w1049, "Time (s)"=w1048) -> (w1045:cluster{"Time (s)":dbl, T3, bool})  [unwired: 2 in]
                n445 = Replace Array Subset(array=w1046, new element=w1045, index=w1044) -> (w1047:cluster{"Time (s)":dbl, T3, bool}[])
              }
            }
          }
        }
        n446 = Sort 1D Array(array=w1012) -> (sorted array=w1011:cluster{"Time (s)":dbl, T3, bool}[])
        n447 = event-data("Discard?"=w1014) -> ()  [unwired: 1 in, 1 out]
        n448 = Not(x=w1014) -> (.not. x?=w1015:bool)
      }
      event "Command Palette": Mouse Move {
        # "Draw the hilite for the row that the mouse is over"
        n449 = event-data() -> ("Coords"=w1057:T31)  [unwired: 1 in]
        n450 = Unbundle(w1060) -> ("Updated Waypoints"=w1059:cluster{"x":dbl, "y":dbl, "th":dbl}[])  [unwired: 3 out]
        n451 = control-ref of="Command Palette"() -> (w1053:refnum<vi>)
        n452 = call "Picture Coord to Row.vi"("Row Height"=w1052, "Coords"=w1057, "Picture in"=w1053) -> ("Row Index"=w1054:i32, "Clicked in canvas"=w1056:bool)  [unwired: 7 in]
        n453 = Unbundle(w1050) -> ("Filtered Command Info Out"=w1055:T2, "2D Picture"=w1058:picture)  [unwired: 1 out]
        n454 = case shown="True" w1056 {
          tunnel: w1058 -> [_ w1068]
          tunnel: w1055 -> [_ _]
          tunnel: w1052 -> [_ w1066]
          tunnel: w1054 -> [_ w1065]
          frame False {
          }
          frame True {
            n455 = Multiply(x=w1065, y=w1066) -> (x*y=w1071:i32)
            n456 = Add(x=w1071, y=w1066) -> (x+y=w1072:i32)
            n457 = Bundle(0, w1071, 300, w1072) -> (w1073:cluster{i32, i32, i32, i32})  [unwired: 1 in]
            n458 = call <vilib>:"Draw Rectangle.vi"("rect"=w1073, "fill?(F)"=TRUE, "color(black)"=u32 10539263) -> ("new picture"=w1075:picture)  [unwired: 6 in]
            n459 = Concatenate Strings(w1075, w1068) -> (→"Command Palette":picture)
          }
        }
      }
      event "Command Palette": Mouse Down {
        # "When a double click occurs in the command palette,\nadd the command to the command list at time T."
        n460 = event-data() -> ("Coords"=w1087:T31, "Mods"=w1089:cluster{"Double Click":bool, "Menu Key":bool})  [unwired: 1 in, 1 out]
        n461 = control-ref of="Command Palette"() -> (w1088:refnum<vi>)
        n462 = Unbundle(w1091) -> ("Updated Waypoints"=w1090:cluster{"x":dbl, "y":dbl, "th":dbl}[])  [unwired: 3 out]
        n463 = call "Picture Coord to Row.vi"("Row Height"=w1086, "Coords"=w1087, "Picture in"=w1088) -> ("Row Index"=w1082:i32, "Clicked in canvas"=w1085:bool)  [unwired: 7 in]
        n464 = Unbundle(w1089) -> ("Double Click"=w1084:bool)  [unwired: 1 out]
        n465 = Unbundle(w1078) -> ("Filtered Command Info Out"=w1081:T2)  [unwired: 2 out]
        n466 = Compound Arithmetic op=AND(w1085, w1084) -> (w1083:bool)
        n467 = case shown="True" w1083 {
          tunnel: w1082 -> [_ w1103]
          tunnel: w1081 -> [_ w1104]
          tunnel: w1080 -> [w1096 w1098]
          tunnel: [w1096 w1099] -> w1077
          frame False {
          }
          frame True {
            n468 = local read "Time (s)"() -> (w1100:dbl)
            n469 = Index Array(array=w1104, index=w1103) -> (element=w1102:T3)
            n470 = Bundle("Time (s)"=w1100, w1102, TRUE) -> (w1097:cluster{"Time (s)":dbl, T3, bool})  [unwired: 1 in]
            n471 = call "Insert Into Sorted Array.vim"("element"=w1097, "sorted array in"=w1098) -> ("sorted array out"=w1099:cluster{"Time (s)":dbl, T3, bool}[])  [unwired: 9 in]
          }
        }
      }
    }
    n472 = feedback-in #1(w98) -> ()
    n473 = Unbundle(w74) -> (w73:T14)  [unwired: 3 out]
    n474 = Unbundle(w73) -> ("Limits"=w75:T9)  [unwired: 4 out]
    n475 = Unbundle(w75) -> ("Velocity (fps)"=w72:dbl)  [unwired: 3 out]
    n476 = flat-sequence {
      tunnel: ["Time (s)"] -> w113
      tunnel: ["Sample Period (s)"] -> w87
      tunnel: ["Limits"] -> w66
      tunnel: ["Conditions"] -> w52
      tunnel: [w128] -> w76
      tunnel: ["Overrides"] -> w51
      tunnel: w80 -> [w128]
      tunnel: w79 -> [w130]
      tunnel: ["Hide Path"] -> w70
      tunnel: ["Stoopid Overlap %"] -> w69
      tunnel: ["Angular Limits"] -> w50
      tunnel: [w122] -> w47
      frame #0 {
        n477 = control-ref of="Command Sequence"() -> (w131:refnum<vi>)
        n478 = global write "Global Settings.vi" "> 90?"("Allow Angles > 90") -> ()
        n479 = global write "Global Settings.vi" "Turn Angle Limit (deg)"("Turn Angle Limit (deg)") -> ()
        n480 = call "Format Tree.vi"("Update"=w130, "Commands"=w128, "Tree Refnum"=w131) -> ()  [unwired: 9 in]
        n481 = local read "Overrides"() -> (w122:T8)
      }
    }
    n482 = Unbundle(w66) -> ("Accel (fps^2)"=w65:dbl)  [unwired: 3 out]
    n483 = Divide(x=w113, y=w87) -> (x/y=w106:dbl)
    n484 = Bundle("Sample Period (s)"=w87, "Limits"=w66, "Conditions"=w52, "Overrides"=w51, "Angular Limits"=w50) -> (w67:T14)  [unwired: 1 in]
    n485 = call "Enforce Robot Rules.vi"("max V"=w72, "Drive Type"="Drive Type", "Overrides"=w47, "turn accel"=w65, "Disable"=w60, "New Points"=w108, "Original Points"=w107) -> ("Overrides Out"=w53:T8, "Points out"=w49:cluster{"x":dbl, "y":dbl, "th":dbl}[])  [unwired: 3 in]
    n486 = call "GenNewTraj.vi"("Drive Type"="Drive Type", "Turn Rate"="Turn Rate", "Stoopid Overlap %"=w69, "Path Type"="Path Type", "Parameters"=w67, "Points in"=w49) -> ("Time & Dist"=w59:cluster{"Time (s)":dbl, "Distance (ft)":dbl}, "Valid"=w44:bool, "Trajectory Data"=w95:T12, "Updated Waypoints"=w99:cluster{"x":dbl, "y":dbl, "th":dbl}[])  [unwired: 2 in]
    "Trajectory Data" <- w95
    n487 = local write "WayPoints"(w49) -> ()
    n488 = local write "Overrides"(w53) -> ()
    n489 = Unbundle(w59) -> ("Time (s)"=w57:dbl, "Distance (ft)"=→"Distance (ft)":dbl)
    "Duration (s)" <- w57
    n490 = Unbundle(w93) -> ("Hover Object"=w92:T17)  [unwired: 2 out]
    n491 = Bundle(cluster=T20 {"Trajectory Data"=[], "Updated Waypoints"=[], {"Sample Period (s)"=0.0, "Limits"={"Velocity (fps)"=0.0, "Accel (fps^2)"=0.0, "Jerk (fps^3)"=0.0, "StoopidFast (fps)"=0.0}, "Conditions"={"vInitial (fps)"=0.0, "vFinal (fps)"=0.0}, "Overrides"=[], "Angular Limits"={"Velocity (deg/s)"=6.0, "Accel (deg/s^2)"=15.0, "Jerk (deg/s^3)"=150.0}}, "Commands out"=[]} ("output cluster"), "Trajectory Data"=w95, "Updated Waypoints"=w99, w67, "Commands out"=w76) -> (w54:T20)
    n492 = property on="Time (s)" class="Slide (strict)"("Scale.Minimum"=0.0 ("Scale.Range:Minimum"), "Scale.Maximum"=w57) -> ()  [unwired: 2 in, 2 out]
    n493 = call "Draw Trajectory.vi"("Robot Index"=w106, "Hide Path"=w70, "new picture in"=picture data[5B] ("new picture"), "Trajectory Data"=w95, "Picture in"=w116) -> ("Path Points"=w100:cluster{"x":dbl, "y":dbl}[], "Output Point"=w112:T39, "new picture"=w114:picture)  [unwired: 4 in]
    n494 = call "Draw Shapes.vi"("Picture in"=w116, "Commands"=w76, "Sample Period (s)"=w87, "Points"=w99, "Valid Path?"=w44, "new picture in"=w114, "Results"=w92, "Output Point"=w112, "Path Points"=w100) -> ("new picture out"=→"Picture":picture)  [unwired: 6 in]
    n495 = call "Update Annotations.vi"("Sample Period"=w87, "Commands"=w76, "Trajectory Data"=w95, "Robot Pt Index"=w106) -> ("Redraw"=w78:bool, "Velocity Trace"=w77:dbl[], "Annotation Data"=w105:T40)  [unwired: 5 in]
    n496 = case shown="True" w78 {
      tunnel: w105 -> [_ w1106]
      tunnel: w77 -> [_ w1105]
      frame False {
      }
      frame True {
        n497 = property on="fps" class="WFGraph (strict)"("AnntList"=w1106) -> ()  [unwired: 2 in, 2 out]
        "fps" <- w1105
      }
    }
    n498 = disable-structure shown="Disabled" {
      disable-tunnel: w44 -> [w119 _]
      frame Disabled {
        n499 = Select(t=cluster{u32, u32}[] [{14869218, 14869218}] ("Colors [4]"), s=w119, f=cluster{u32, u32}[] [{6094681, 6094681}] ("Colors [4]")) -> ()  [unwired: 1 out]
      }
      frame Enabled {
      }
    }
    n500 = control-ref of="Save"() -> (w63:refnum<vi>)
    n501 = Select(t=0, s=w88, f=2000) -> (s? t:f=w89:i32)
    n502 = call "Saved Checker.vi"("comp B"=w101, "comp A"=w54, "Save button ref"=w63) -> ()  [unwired: 1 in]
  }
  n503 = local write "Time (s)"(0.0 ("Time")) -> ()
